vi "ConvertGoop2ToGoop3.vi"() -> (0 "error out":errorcluster)   [LabVIEW 2020]
uses:
  ConvertGoop2ToGoop3_SubVIs/ConvertGoop2ToGoop3_ClassInfo.ctl
  LvClass_class/GDSLvCLass_ClassSettingsType.ctl
  LvClass_class/GDSLvClass_PlugIn.ctl
  LvClass_class/GDSLvClass_PlugInTypes.ctl
  <vilib>/Utility/miscctls.llb/LVPositionTypeDef.ctl
  <vilib>/Utility/error.llb/DialogType.ctl
  <vilib>/picture/picture.llb/imagedata.ctl
  Provider_EndevoGOOP300/Templates/EndevoTemplateNames.ctl
  Provider_EndevoGOOP300/EndevoProviderName.ctl
  <vilib>/regexp/Match Regular Expression.xnode
panel:
  in  "Cancel":bool
  in  "Next":bool
  out "Tab":T1(tab)
  in  "Current GOOP2 top directory":path
  out "Additional VIs that has been found\nand will be relinked:":i32
  out "GOOP2 classes found":string
  in  "VisToRelink":path[](array[path])
  in  "Project":path caption="This project will be created and have all classes added to it:"
  in  "Progress":i32(listbox)
  in  "Done":bool
  out "State":string
  # "1."
  # "Select Top folder to start a recursive search for GOOP2 classes and application VIs."
  # "2."
  # "These classes\nhave been found.\n\nDo you want to convert them?"
  # "3."
  # "Have you backed up all your VIs in the selected folder?"
  # "Have you checked that all files in\nthe selected folder are writeable?"
  # "Relinking VIs outside top folder?\nIf you want to relink any VIs to the new classes that are outside the selected top folder, add them to the list below"
  # "4."
  # "Save VI dialog boxes!?!\nIt might pop up dialog boxes that asks you to save VIs that will be unloaded from memory, JUST press cancel for those."
  # "5."
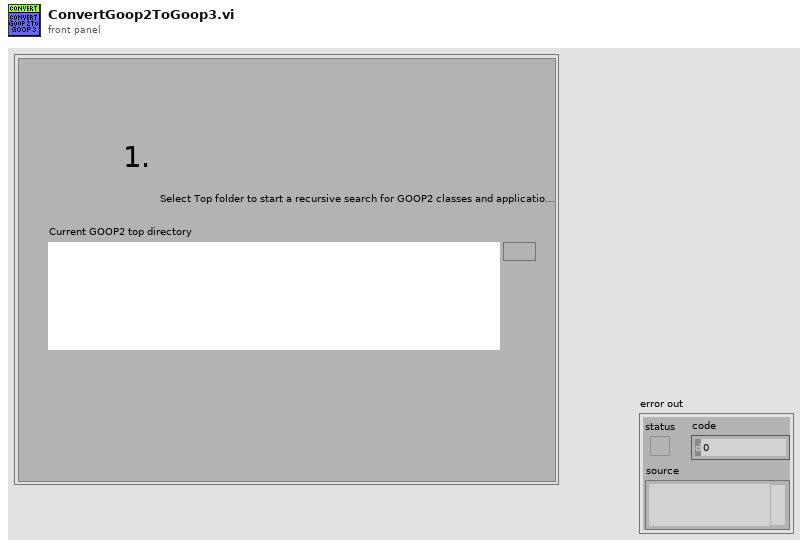
[diagram p1: front panel]
types:
  T1 = enum32{"GOOP2Dir", "ClassesFound", "BackedUp", "Start?", "Converting"}
  T2 = typedef "ConvertGoop2ToGoop3_ClassInfo.ctl" = cluster{"NoOfInheritance":i32, "LvClassPath":path, "ClassName":string, "ClassPrefix":string, "IsLLB":bool, "ClassFolder":path, "ViRefs":refnum<vi>[], "ClassRef":refnum<vi>, "InheritsFrom":path, "RootClass":path, "ViPathes":path[], "AllInheritanceClasses":string[], "TemplateVersionUsed":string, "UsingClassAttributes":bool, "ClassSettings":T3, "HeaderIcon":u8[][]}
  T3 = typedef "GDSLvCLass_ClassSettingsType.ctl" = cluster{"ClassProviderName":string, "ClassTemplateUsed":string, "ClassTemplateVersion":string, "ClassDescription":string, "PlugIns":T4[], "ConnectorPanePattern":string}
  T4 = typedef "GDSLvClass_PlugIn.ctl" = cluster{"Type":T5, "ID":string, "Version":string, "Path":path, "Name":string, "Data":variant}
  T5 = typedef "GDSLvClass_PlugInTypes.ctl" = enum16{"DesignPattern", "MethodTypes"}
  T6 = typedef "LVPositionTypeDef.ctl" = cluster{"Left":i32, "Top":i32}
  T7 = cluster{"TopFolderPath":path, "Classes":T2[], "SetToDynamicDispatch":refnum<vi>[], "error":errorcluster, "Project":path, "ProjectRef":refnum<vi>, "My Computer":refnum<vi>, "AppRef":refnum<vi>, "VIsToRelink":refnum<vi>[], "VIsToRelink(Paths)":path[], "CallParentMethod":cluster{"VIRef":refnum<vi>, "Position":T6}[], "TemplateVersionUsed":string}
  T8 = enum32{"GOOP2Dir", "ClassesFound", "GOOP3Dir", "Start?", "Converting"}
  T9 = typedef "imagedata.ctl" = cluster{"image type":i32, "image depth":i32, "image":u8[], "mask":u8[], "colors":u32[], "Rectangle":cluster{"left":i16, "top":i16, "right":i16, "bottom":i16}}
  T10 = typedef "EndevoTemplateNames.ctl" = enum16{"BaseTemplate", "SubTemplate", "BaseTemplate_4x4x4", "SubTemplate_4x4x4", "SingletonTemplate"}
  T11 = typedef "EndevoProviderName.ctl" = enum16{"EndevoGOOP300"}
  T12 = typedef "DialogType.ctl" = u16
  T13 = enum32{"invalid VI type", "Standard VI", "Control VI", "Global VI", "Polymorphic VI", "Configuration VI", "SubSystem", "Facade VI", "Method VI", "Statechart Diagram VI"}
  T14 = enum16{"Invalid Wire Rule", "Required", "Recommended", "Optional", "Dynamic Dispatch"}
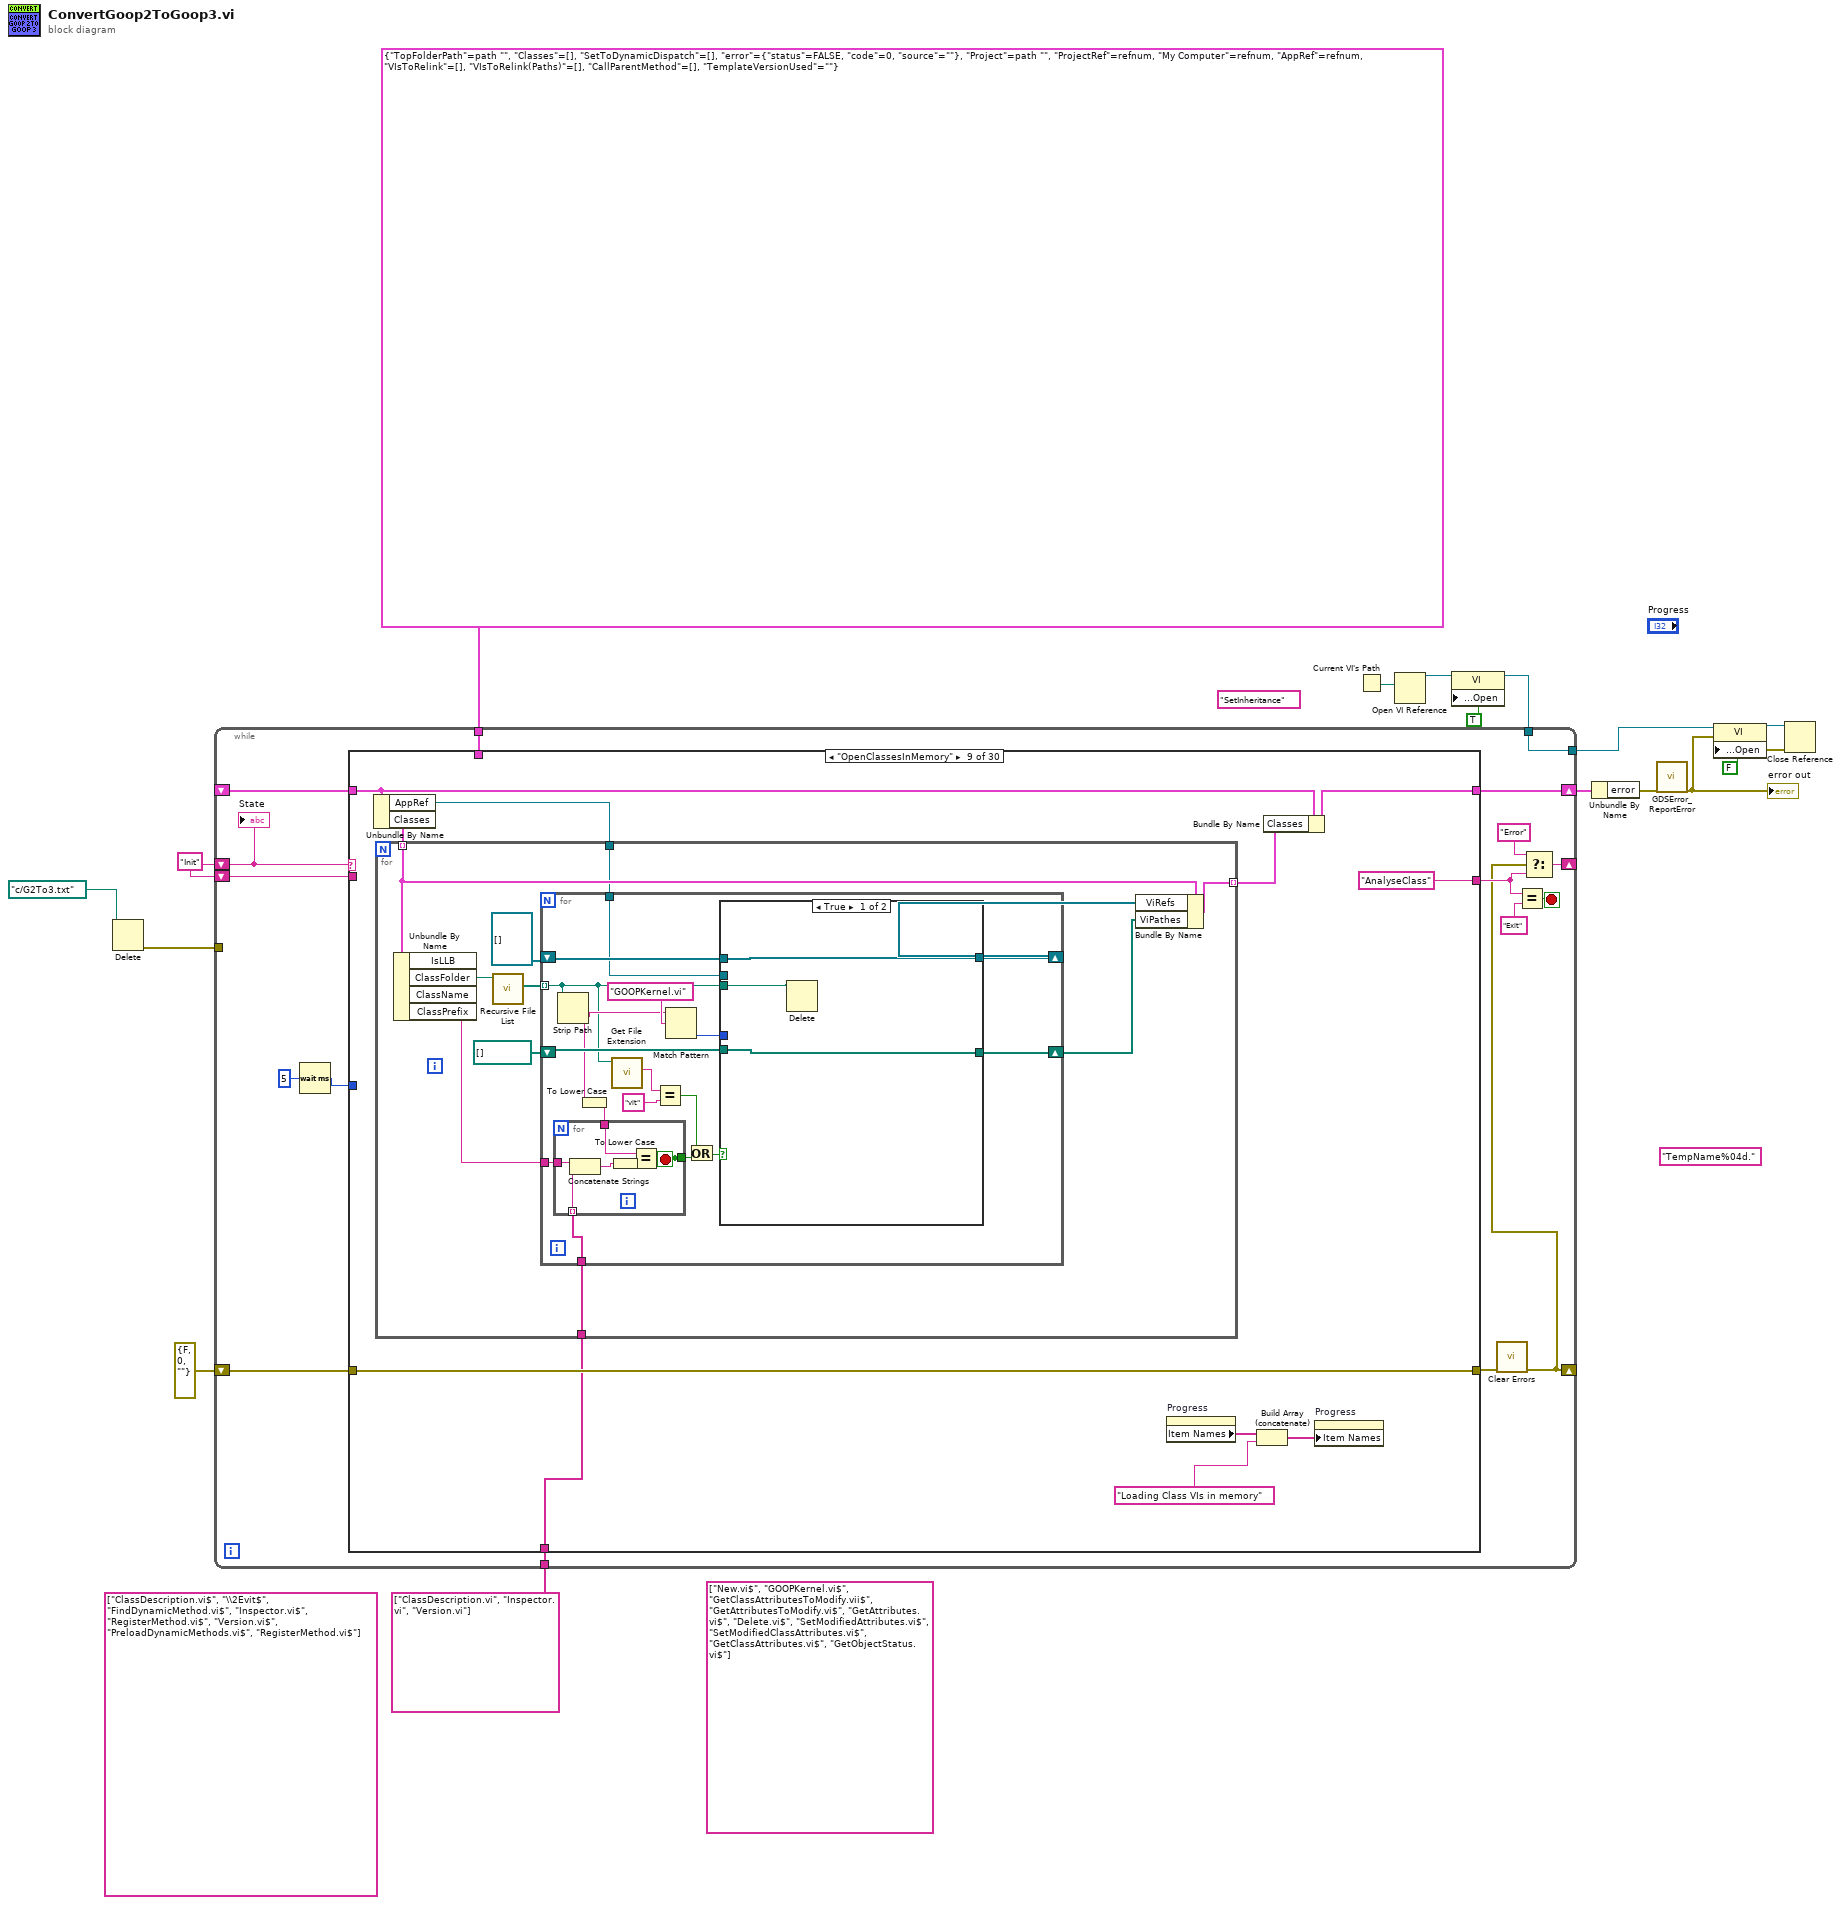
[diagram p0: block diagram]
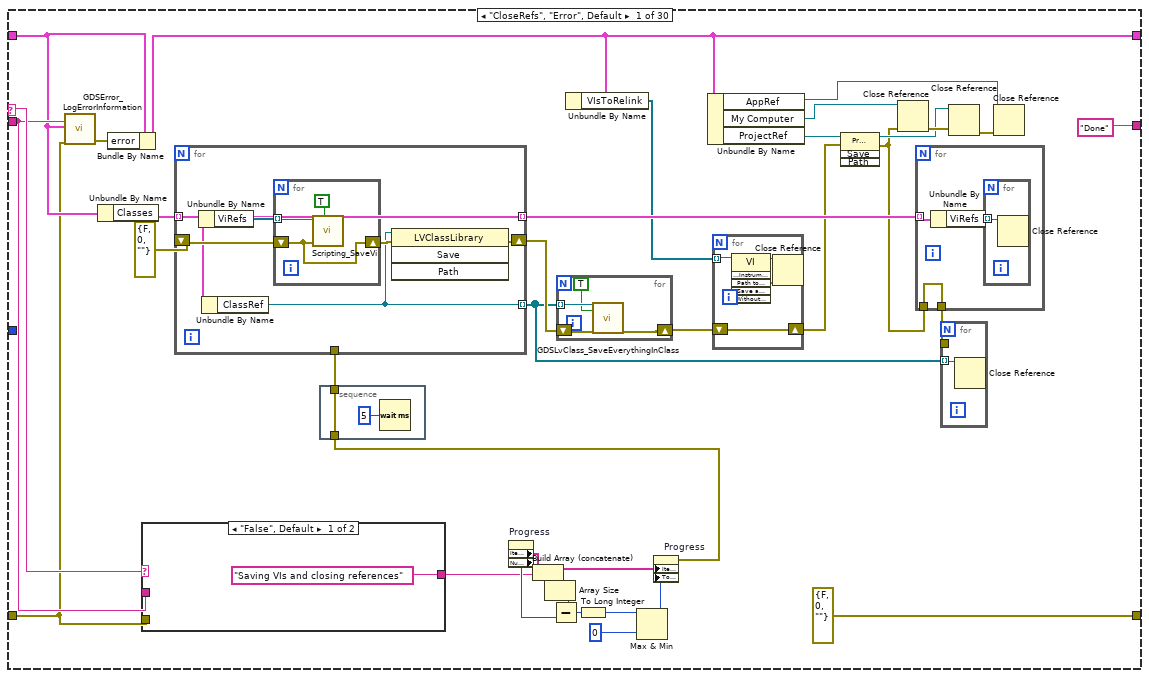
[diagram p2: hidden frame]
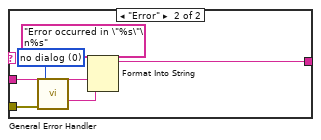
[diagram p3: hidden frame]
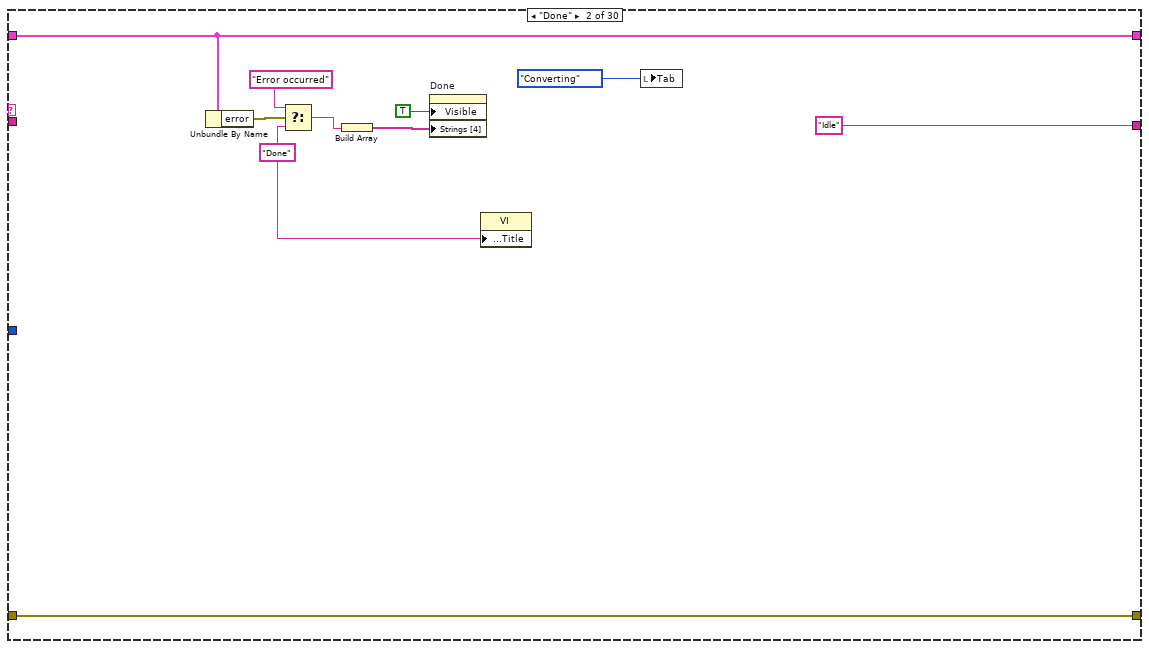
[diagram p4: hidden frame]
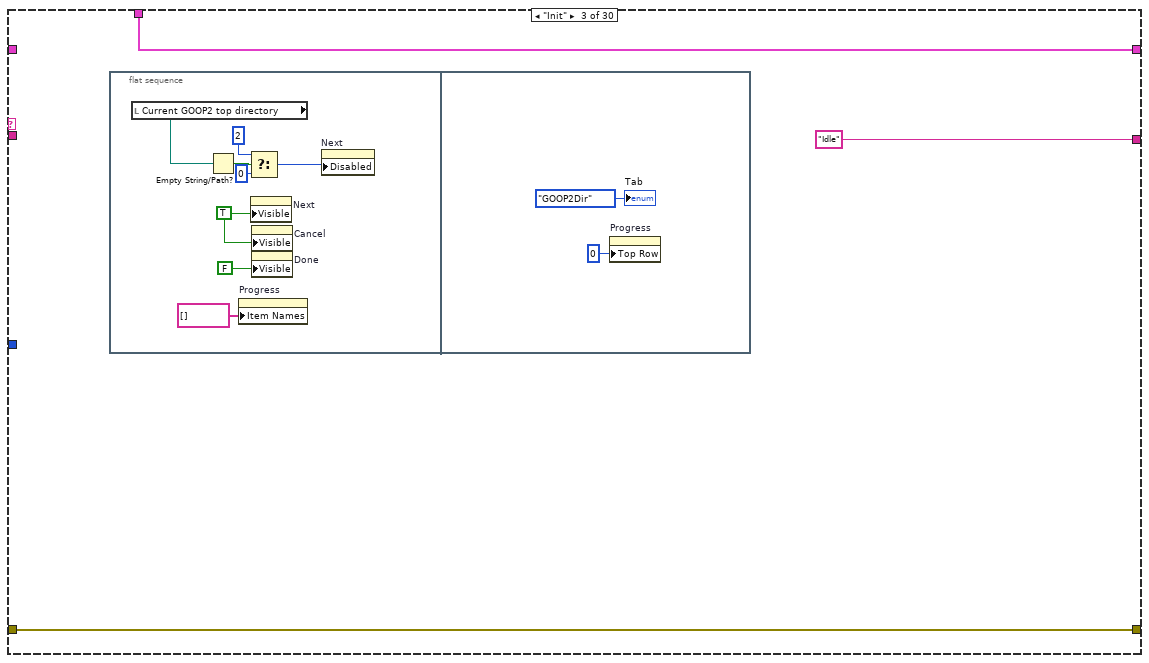
[diagram p5: hidden frame]
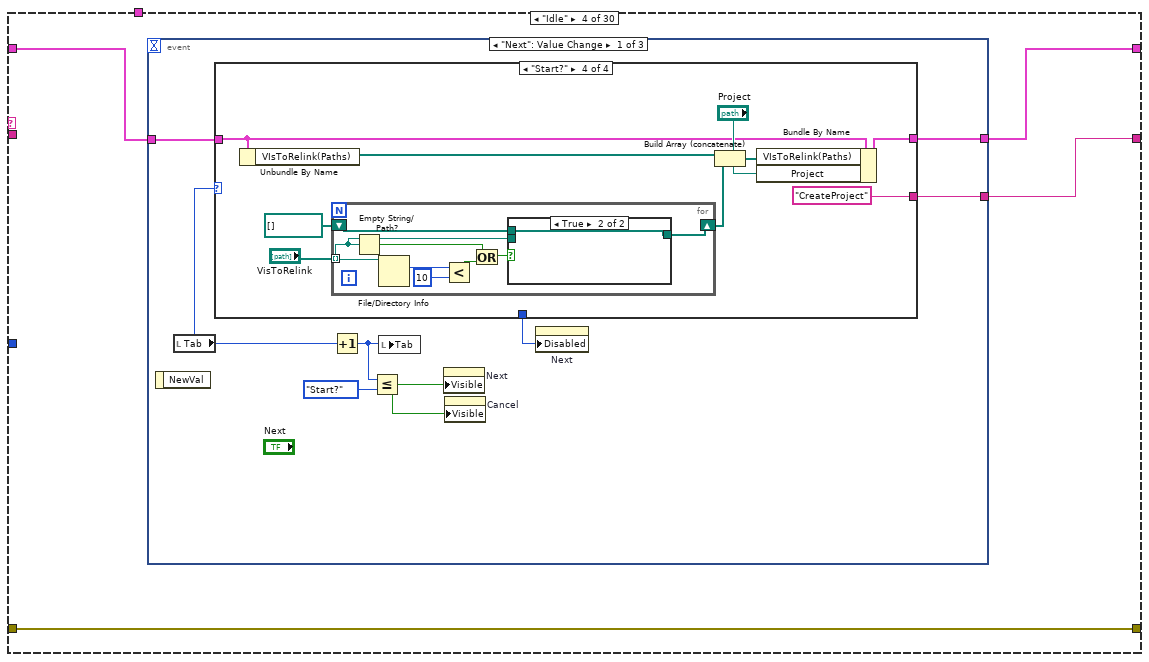
[diagram p6: hidden frame]
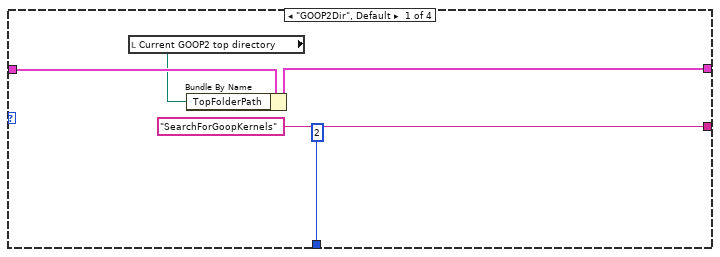
[diagram p7: hidden frame]
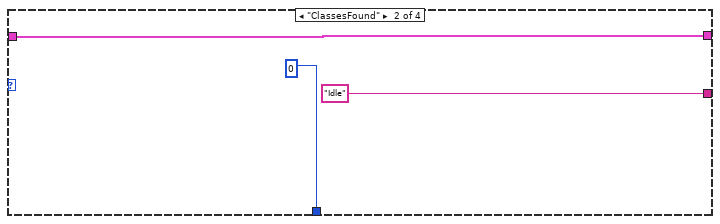
[diagram p8: hidden frame]
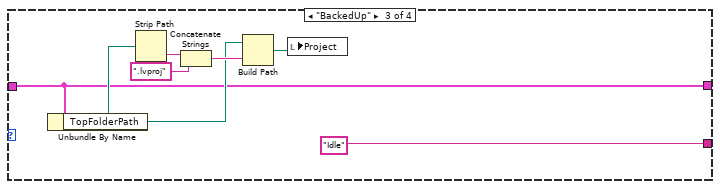
[diagram p9: hidden frame]
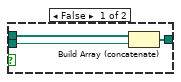
[diagram p10: hidden frame]
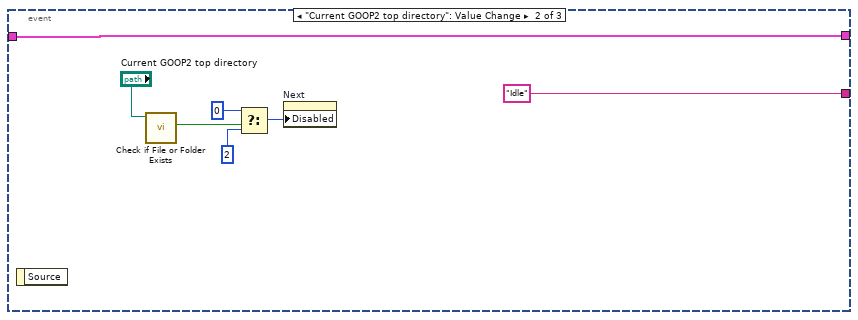
[diagram p11: hidden frame]
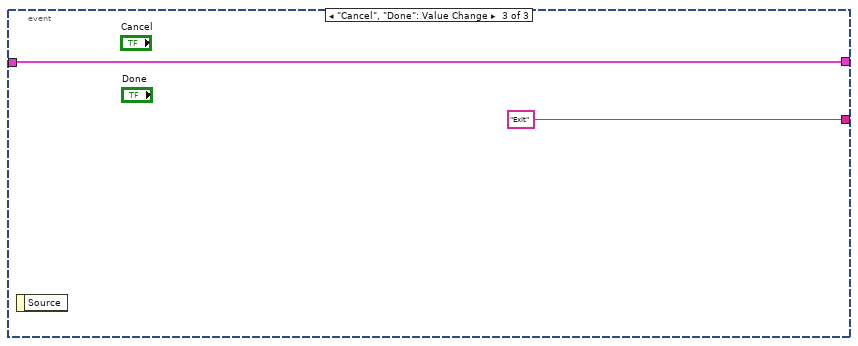
[diagram p12: hidden frame]
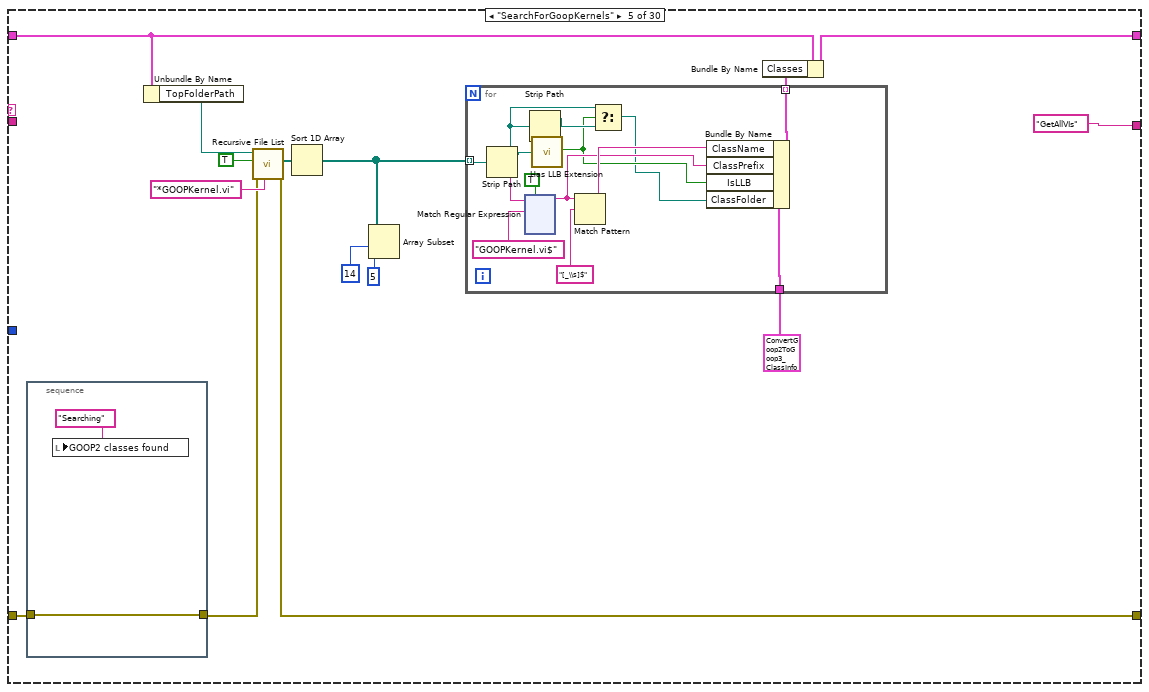
[diagram p13: hidden frame]
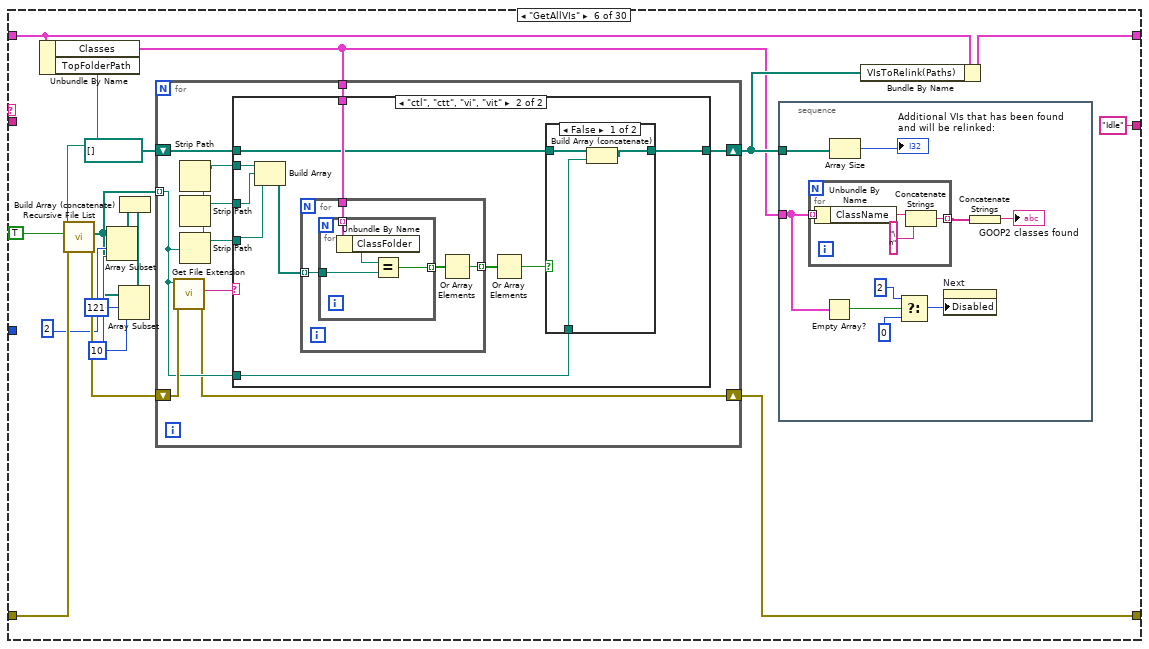
[diagram p14: hidden frame]
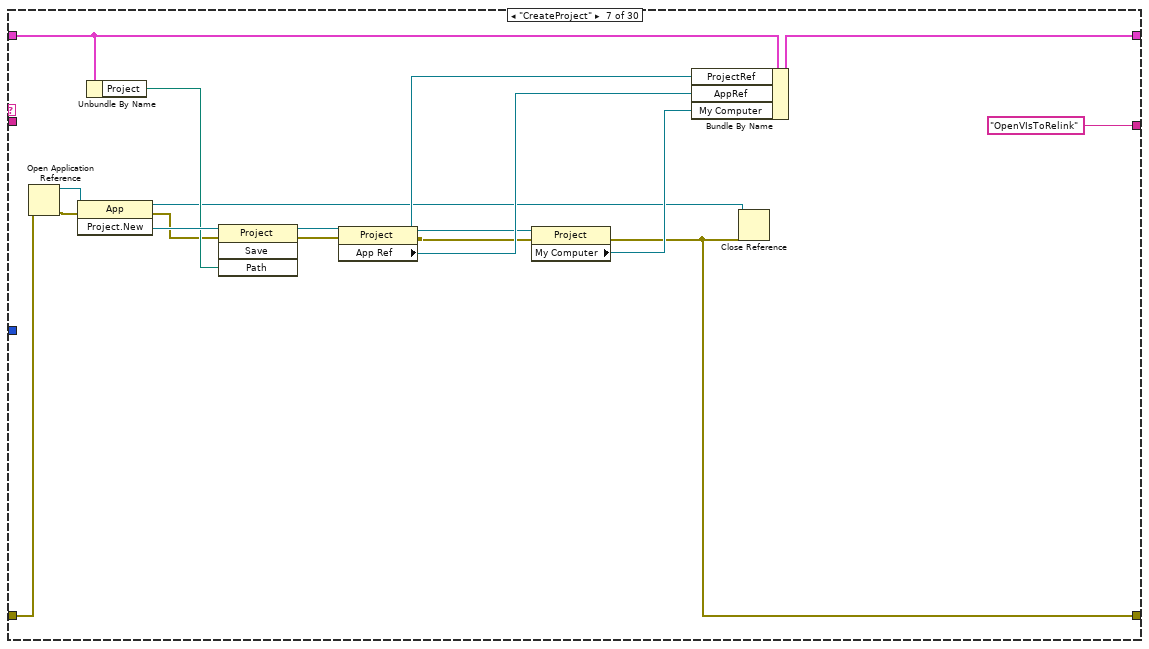
[diagram p17: hidden frame]
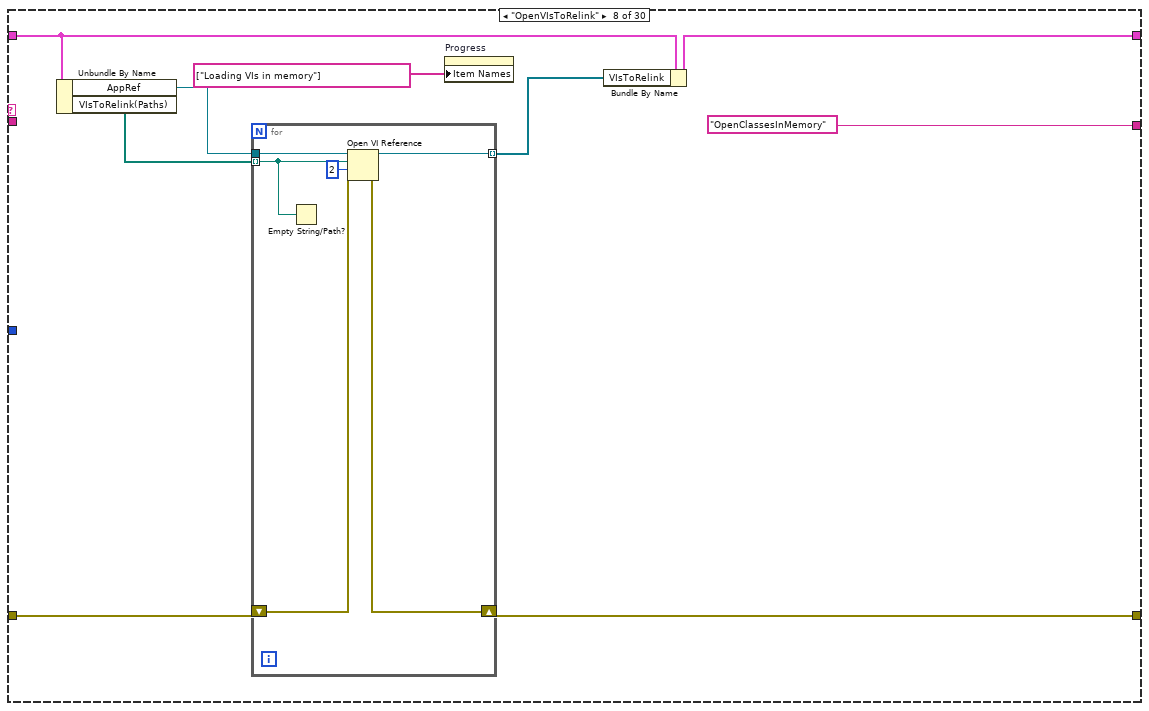
[diagram p18: hidden frame]
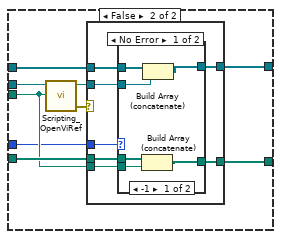
[diagram p19: hidden frame]
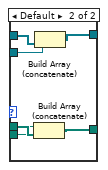
[diagram p20: hidden frame]
diagram:
  (unwired) "SetInheritance"
  (unwired) "TempName%04d." ("format string")
  (unwired) string[] ["ClassDescription.vi$", "\\2Evit$", "FindDynamicMethod.vi$", "Inspector.vi$", "RegisterMethod.vi$", "Version.vi$", "PreloadDynamicMethods.vi$", "RegisterMethod.vi$"] ("file names")
  (unwired) string[] ["New.vi$", "GOOPKernel.vi$", "GetClassAttributesToModify.vii$", "GetAttributesToModify.vi$", "GetAttributes.vi$", "Delete.vi$", "SetModifiedAttributes.vi$", "SetModifiedClassAttributes.vi$", "GetClassAttributes.vi$", "GetObjectStatus.vi$"] ("file names")
  w15 = "Init"
  n1 = Delete(path (use dialog)=path "c:/G2To3.txt" ("file (use dialog)")) -> (error out=w12:errorcluster)  [unwired: 4 in, 2 out]
  n2 = Current VI's Path() -> (path=w10:path)
  n3 = Open VI Reference(vi path=w10) -> (vi reference=w8:refnum<vi>)  [unwired: 5 in, 1 out]
  n4 = property class="VI"(reference=w8, "Front Panel.Open"=TRUE ("Front Panel Window:Open")) -> (reference out=w7:refnum<vi>)  [unwired: 1 in, 1 out]
  n5 = while {
    shift-right: [w19] -> _
    shift-left: errorcluster {"status"=FALSE, "code"=0, "source"=""} ("error IO") -> [w34]
    shift-right: [w33] -> _
    shift-left: w15 -> [w24]
    shift-right: [w28] -> w14
    shift-left: _ -> [w27]
    tunnel: T7 {"TopFolderPath"=path "", "Classes"=[], "SetToDynamicDispatch"=[], "error"={"status"=FALSE, "code"=0, "source"=""}, "Project"=path "", "ProjectRef"=refnum, "My Computer"=refnum, "AppRef"=refnum, "VIsToRelink"=[], "VIsToRelink(Paths)"=[], "CallParentMethod"=[], "TemplateVersionUsed"=""} -> [w26]
    shift-left: w15 -> [w25]
    tunnel: w12 -> [_]
    tunnel: w7 -> [w21]
    tunnel: [w21] -> w5
    tunnel: string[] ["ClassDescription.vi", "Inspector.vi", "Version.vi"] ("file names") -> [w18]
    stop <- w32 stop-if-true
    n6 = Wait (ms)(milliseconds to wait=u32 5) -> (millisecond timer value=w22:u32)
    n7 = case shown="\"OpenClassesInMemory\"" w24 {
      selector: w24 -> [w64 _ _ _ _ _ _ _ _ _ _ _ _ _ _ _ _ _ _ _ _ _ _ _ _ _ _ _ _ _]
      tunnel: w34 -> [w58 w109 w112 w124 w188 w335 w395 w407 w423 w504 w533 w576 w586 w625 w757 w799 w883 w929 w981 w1030 w1071 w1158 w1220 w1277 w1329 w1409 w1423 w1481 w1515 w1559]
      tunnel: [errorcluster {"status"=FALSE, "code"=0, "source"=""} ("error IO") w109 w112 w124 w192 w333 w386 w406 w423 w504 w532 w574 w582 w626 w760 w798 w894 w931 w982 w1032 w1065 w1145 w1213 w1274 w1335 w1408 w1423 w1482 w1510 w1547] -> w20
      tunnel: ["Done" "Idle" "Idle" w125 "GetAllVIs" "Idle" "OpenVIsToRelink" "OpenClassesInMemory" "AnalyseClass" "RemoveReentrantForDynamicDispatchVIs" "RecompilingVIs" "AddVIsToProject" "RenameFiles" "RenameTempNames" "FindAllCallParentMethodCalls" "UpdateNewVI" "SetInheritance" "UpdateLvClassIcon" "UpdateLvClassAttributes" "UpdateUtilsVIs" "UpdateSubClassKernels" "UpdateVIsGoopRefs" "UpdateCreate" "UpdateDynamicDispatchVIs" "ExtraSave" "SetDynamicDispatch" "UpdateAllCallParentMethods" "UpdateDestroy" "UpdateClassInfo" "CloseRefs"] -> w29
      tunnel: [w47 w108 w111 w126 w190 w331 w397 w409 w425 w502 w534 w575 w579 w624 w758 w796 w881 w930 w984 w1031 w1067 w1144 w1212 w1271 w1332 w1407 w1422 w1479 w1514 w1558] -> w28
      tunnel: w27 -> [w60 w108 _ w127 w191 w332 w399 w410 w426 w503 w534 w575 w579 w619 w758 w797 w881 w930 w984 w1031 w1064 w1144 w1212 w1271 w1327 w1407 w1422 w1479 w1514 w1558]
      tunnel: w26 -> [_ _ w111 _ _ _ _ _ _ _ _ _ _ _ _ _ _ _ _ _ _ _ _ _ _ _ _ _ _ _]
      tunnel: w25 -> [w63 _ _ _ _ _ _ _ _ _ _ _ _ _ _ _ _ _ _ _ _ _ _ _ _ _ _ _ _ _]
      tunnel: w22 -> [_ _ _ _ _ _ _ _ _ _ _ _ _ _ _ _ _ _ _ _ _ _ _ _ _ _ _ _ _ _]
      tunnel: w18 -> [_ _ _ _ _ _ _ _ w417 _ _ _ _ _ _ _ _ _ _ _ _ _ _ _ _ _ _ _ _ _]
      frame "CloseRefs", "Error", Default {
        n8 = call "GDSError_LogErrorInformation.vi"("State"=w63, "LocalVariableData"=w60, "error in (no error)"=w58) -> ("error out"=w50:errorcluster)  [unwired: 16 in]
        n9 = Unbundle By Name(w60) -> ("Classes"=w68:T2[])
        n10 = Bundle By Name(cluster=w60, "error"=w50) -> (w47:T7)
        n11 = case shown="\"False\", Default" w64 {
          tunnel: w63 -> [_ w81]
          tunnel: w58 -> [_ w79]
          tunnel: ["Saving VIs and closing references" w77] -> w37
          frame "False", Default {
          }
          frame "Error" {
            w80 = T12 0 items=["no dialog", "OK message", "continue or stop message", "OK message + warnings", "continue/stop + warnings"] ("type of dialog (OK msg:1)")
            n12 = call <vilib>:"General Error Handler.vi"("type of dialog (OK msg:1)"=w80, "error in (no error)"=w79) -> ("message"=w78:string)  [unwired: 9 in, 4 out]
            n13 = Format Into String(format string="Error occurred in \"%s\"\n%s", w81, w78) -> (resulting string=w77:string)  [unwired: 2 in, 1 out]
          }
        }
        n14 = property on="Progress" class="LstBox (strict)"() -> ("Item Names"=w45:string[], "Number of Rows"=w39:u32)  [unwired: 2 in, 2 out]
        n15 = Build Array (concatenate)(w45, w37) -> (w40:string[])
        n16 = Array Size(array=w40) -> (size(s)=w44:i32)
        n17 = Subtract(x=w44, y=w39) -> (x-y=w43:u32)
        n18 = Unbundle By Name(w47) -> ("VIsToRelink"=w52:refnum<vi>[])
        n19 = To Long Integer(number=w43) -> (32bit integer=w41:i32)
        n20 = Max & Min(x=w41, y=0) -> (max(x,y)=w38:i32)  [unwired: 1 out]
        n21 = property on="Progress" class="LstBox (strict)"("Item Names"=w40, "Top Row"=w38) -> (error out=w36:errorcluster)  [unwired: 2 in, 1 out]
        n22 = stacked-sequence {
          tunnel: w36 -> [w70]
          tunnel: [w70] -> w35
          frame #0 {
            n23 = Wait (ms)(milliseconds to wait=u32 5) -> ()  [unwired: 1 out]
          }
        }
        n24 = for {
          tunnel: w68 -> [w95] mode=indexing
          tunnel: [w95] -> w67 mode=indexing
          shift-right: [w93] -> w66
          shift-left: errorcluster {"status"=FALSE, "code"=0, "source"=""} ("error out") -> [w96]
          tunnel: [w92] -> w65 mode=indexing
          tunnel: w35 -> [_]
          n25 = Unbundle By Name(w95) -> ("ViRefs"=w97:refnum<vi>[])
          n26 = Unbundle By Name(w95) -> ("ClassRef"=w92:refnum<vi>)
          n27 = for {
            tunnel: w97 -> [w100] mode=indexing
            shift-right: [w98] -> w94
            shift-left: w96 -> [w98]
            n28 = call "Scripting_SaveVi.vi"("ForceResaving(False)"=TRUE, "error in (no error)"=w98, "VIRefToSaveIn"=w100) -> ()  [unwired: 7 in, 2 out]
          }
          n29 = invoke class="LVClassLibrary" method="Save"(reference=w92, error in=w94) -> (error out=w93:errorcluster)  [unwired: 2 in, 3 out]
        }
        n30 = for {
          shift-right: [w86] -> w49
          shift-left: w66 -> [w87]
          tunnel: w65 -> [w85] mode=indexing
          n31 = call "GDSLvClass_SaveEverythingInClass.vi"("ClassRefIn"=w85, "ForceResaving(False)"=TRUE, "error in"=w87) -> ("error out"=w86:errorcluster)  [unwired: 15 in, 1 out]
        }
        n32 = Unbundle By Name(w47) -> ("AppRef"=w53:refnum<vi>, "My Computer"=w46:refnum<vi>, "ProjectRef"=w57:refnum<vi>)
        n33 = for {
          tunnel: w52 -> [w73] mode=indexing
          shift-right: [w72] -> w48
          shift-left: w49 -> [w72]
          n34 = invoke class="VI" method="Save.Instrument"(reference=w73) -> (reference out=w74:refnum<vi>, error out=w75:errorcluster)  [unwired: 5 in, 4 out]
          n35 = Close Reference(reference=w74, error in (no error)=w75) -> ()  [unwired: 1 out]
        }
        n36 = invoke class="Project" method="Save"(reference=w57, error in=w48) -> (reference out=w55:refnum<vi>, error out=w51:errorcluster)  [unwired: 2 in, 2 out]
        n37 = Close Reference(reference=w46, error in (no error)=w51) -> (error out=w56:errorcluster)
        n38 = for {
          tunnel: w67 -> [w90] mode=indexing
          tunnel: w51 -> [w88]
          tunnel: [w88] -> w62
          n39 = Unbundle By Name(w90) -> ("ViRefs"=w89:refnum<vi>[])
          n40 = for {
            tunnel: w89 -> [w91] mode=indexing
            n41 = Close Reference(reference=w91) -> ()  [unwired: 1 in, 1 out]
          }
        }
        n42 = for {
          tunnel: w65 -> [w83] mode=indexing
          tunnel: w62 -> [_]
          n43 = Close Reference(reference=w83) -> ()  [unwired: 1 in, 1 out]
        }
        n44 = Close Reference(reference=w55, error in (no error)=w56) -> (error out=w54:errorcluster)
        n45 = Close Reference(reference=w53, error in (no error)=w54) -> ()  [unwired: 1 out]
      }
      frame "Done" {
        w101 = "Done"
        n46 = Unbundle By Name(w108) -> ("error"=w107:errorcluster)
        n47 = Select(t="Error occurred", s=w107, f=w101) -> (s? t:f=w104:string)
        n48 = Build Array(w104) -> (w103:string[])
        n49 = property on="Done" class="Bool"("Visible"=TRUE, "Strings [4]"=w103) -> ()  [unwired: 2 in, 2 out]
        n50 = property class="VI"("Front Panel.Title"=w101) -> ()  [unwired: 2 in, 2 out]
        n51 = local write "Tab"(T1."Converting" ("Tab")) -> ()
      }
      frame "Init" {
        n52 = flat-sequence {
          frame #0 {
            w121 = TRUE ("Visible")
            n53 = local read "Current GOOP2 top directory"() -> (w118:path)
            n54 = Empty String/Path?(string/path=w118) -> (empty?=w117:bool)
            n55 = property on="Progress" class="LstBox (strict)"("Item Names"=string[] []) -> ()  [unwired: 2 in, 2 out]
            n56 = Select(t=u8 2 ("Disabled"), s=w117, f=u8 0) -> (s? t:f=w115:u8)
            n57 = property on="Next" class="Bool"("Visible"=w121) -> ()  [unwired: 2 in, 2 out]
            n58 = property on="Cancel" class="Bool"("Visible"=w121) -> ()  [unwired: 2 in, 2 out]
            n59 = property on="Done" class="Bool"("Visible"=FALSE) -> ()  [unwired: 2 in, 2 out]
            n60 = property on="Next" class="Bool"("Disabled"=w115) -> ()  [unwired: 2 in, 2 out]
          }
          frame #1 {
            n61 = property on="Progress" class="LstBox (strict)"("Top Row"=0) -> ()  [unwired: 2 in, 2 out]
            "Tab" <- T1."GOOP2Dir" ("Tab")
          }
        }
      }
      frame "Idle" {
        n62 = event shown="[0] \"Next\": Value Change" {
          selector: _ -> [_ _ _]
          dyn-events: _ -> [_ _ _]
          timeout: _ -> [_ _ _]
          tunnel: w127 -> [w131 w174 w179]
          tunnel: [w130 w174 w179] -> w126
          tunnel: [w129 "Idle" "Exit"] -> w125
          event "Next": Value Change {
            n63 = event-data() -> ()  [unwired: 1 in, 1 out]
            n64 = local read "Tab"() -> (w132:T1)
            n65 = case shown="\"Start?\"" w132 {
              tunnel: w131 -> [w140 w142 w145 w156]
              tunnel: [w139 w142 w145 w159] -> w130
              tunnel: ["SearchForGoopKernels" "Idle" "Idle" "CreateProject"] -> w129
              tunnel: [u8 2 ("Disabled") u8 0 ("f") _ _] -> w128
              frame "GOOP2Dir", Default {
                n66 = local read "Current GOOP2 top directory"() -> (w137:path)
                n67 = Bundle By Name(cluster=w140, "TopFolderPath"=w137) -> (w139:T7)
              }
              frame "ClassesFound" {
              }
              frame "BackedUp" {
                n68 = Unbundle By Name(w145) -> ("TopFolderPath"=w146:path)
                n69 = Strip Path(path=w146) -> (name=w149:string)  [unwired: 1 out]
                n70 = Concatenate Strings(w149, ".lvproj" ("string")) -> (w147:string)
                n71 = Build Path(base path=w146, name or relative path=w147) -> (appended path=w144:path)
                n72 = local write "Project"(w144) -> ()
              }
              frame "Start?" {
                n73 = Unbundle By Name(w156) -> ("VIsToRelink(Paths)"=w155:path[])
                n74 = for {
                  tunnel: "VisToRelink" -> [w161] mode=indexing
                  shift-right: [w160] -> w151
                  shift-left: path[] [] -> [w162]
                  n75 = Empty String/Path?(string/path=w161) -> (empty?=w164:bool)
                  n76 = File/Directory Info(path=w161) -> (size=w167:i64)  [unwired: 1 in, 6 out]
                  n77 = Less?(x=w167, y=i64 10) -> (x < y?=w165:bool)
                  n78 = Or(x=w164, y=w165) -> (x .or. y?=w163:bool)
                  n79 = case shown="True" w163 {
                    tunnel: w162 -> [w170 w171]
                    tunnel: w161 -> [w169 _]
                    tunnel: [w168 w171] -> w160
                    frame False {
                      n80 = Build Array (concatenate)(w170, w169) -> (w168:path[])
                    }
                    frame True {
                    }
                  }
                }
                n81 = Build Array (concatenate)(w155, w151) -> (w154:path[])
                n82 = Bundle By Name(cluster=w156, "VIsToRelink(Paths)"=w154, "Project"="Project") -> (w159:T7)
              }
            }
            n83 = Increment(x=w132) -> (x+1=w135:T1)
            n84 = Less Or Equal?(x=w135, y=T8."Start?") -> (x <= y?=w133:bool)
            n85 = local write "Tab"(w135) -> ()
            n86 = property on="Next" class="Bool"("Visible"=w133) -> ()  [unwired: 2 in, 2 out]
            n87 = property on="Cancel" class="Bool"("Visible"=w133) -> ()  [unwired: 2 in, 2 out]
            n88 = property on="Next" class="Bool"("Disabled"=w128) -> ()  [unwired: 2 in, 2 out]
          }
          event "Current GOOP2 top directory": Value Change {
            n89 = event-data() -> ()  [unwired: 1 in, 1 out]
            n90 = call <vilib>:"Check if File or Folder Exists.vi"("path"="Current GOOP2 top directory") -> ("file or folder exists?"=w178:bool)  [unwired: 8 in, 2 out]
            n91 = Select(t=u8 0, s=w178, f=u8 2 ("Disabled")) -> (s? t:f=w177:u8)
            n92 = property on="Next" class="Bool"("Disabled"=w177) -> ()  [unwired: 2 in, 2 out]
          }
          event "Cancel", "Done": Value Change {
            n93 = event-data() -> ()  [unwired: 1 in, 1 out]
          }
        }
      }
      frame "SearchForGoopKernels" {
        n94 = stacked-sequence {
          tunnel: w188 -> [w196]
          tunnel: [w196] -> w187
          frame #0 {
            n95 = local write "GOOP2 classes found"("Searching" ("GOOP2 classes found")) -> ()
          }
        }
        n96 = Unbundle By Name(w191) -> ("TopFolderPath"=w195:path)
        n97 = call <vilib>:"Recursive File List.vi"("pattern"="*GOOPKernel.vi", "error in (no error)"=w187, "Treat LLBs as Folders?"=TRUE, "Folder Path"=w195) -> ("error out"=w192:errorcluster, "All Files in Dir"=w186:path[])  [unwired: 3 in, 3 out]
        n98 = Sort 1D Array(array=w186) -> (sorted array=w182:path[])
        n99 = Array Subset(array=w182, index=14, length=5) -> ()  [unwired: 1 out]
        n100 = for {
          tunnel: w182 -> [w210] mode=indexing
          tunnel: T2 {"NoOfInheritance"=0, "LvClassPath"=path "", "ClassName"="", "ClassPrefix"="", "IsLLB"=FALSE, "ClassFolder"=path "", "ViRefs"=[], "ClassRef"=refnum, "InheritsFrom"=path "", "RootClass"=path "", "ViPathes"=[], "AllInheritanceClasses"=[], "TemplateVersionUsed"="", "UsingClassAttributes"=FALSE, "ClassSettings"={"ClassProviderName"="", "ClassTemplateUsed"="", "ClassTemplateVersion"="", "ClassDescription"="", "PlugIns"=[], "ConnectorPanePattern"=""}, "HeaderIcon"=[]} ("output cluster") -> [w203]
          tunnel: [w198] -> w181 mode=indexing
          n101 = Strip Path(path=w210) -> (stripped path=w205:path, name=w209:string)
          n102 = xnode "Match Regular Expression"("input string"=w209, "regular expression"="GOOPKernel.vi$", "ignore case? (F)"=TRUE) -> ("before match"=w201:string)  [unwired: 3 in, 4 out]
          n103 = Strip Path(path=w205) -> (stripped path=w204:path)  [unwired: 1 out]
          n104 = call <vilib>:"Has LLB Extension.vi"("path"=w205) -> ("path to VI library?"=w200:bool)
          n105 = Match Pattern(string=w201, regular expression="[_\\s]$") -> (before substring=w202:string)  [unwired: 1 in, 3 out]
          n106 = Select(t=w205, s=w200, f=w204) -> (s? t:f=w199:path)
          n107 = Bundle By Name(cluster=w203, "ClassName"=w202, "ClassPrefix"=w201, "IsLLB"=w200, "ClassFolder"=w199) -> (w198:T2)
        }
        n108 = Bundle By Name(cluster=w191, "Classes"=w181) -> (w190:T7)
      }
      frame "GetAllVIs" {
        w326 = 10 ("length")
        n109 = Unbundle By Name(w332) -> ("Classes"=w329:T2[], "TopFolderPath"=w338:path)
        n110 = call <vilib>:"Recursive File List.vi"("error in (no error)"=w335, "Treat LLBs as Folders?"=TRUE, "Folder Path"=w338) -> ("error out"=w334:errorcluster, "All Files in Dir"=w322:path[])  [unwired: 4 in, 3 out]
        n111 = Array Subset(array=w322, index=2, length=w326) -> (w324:path[])
        n112 = Array Subset(array=w322, index=121, length=w326) -> (w323:path[])
        n113 = Build Array (concatenate)(w324, w323) -> ()  [unwired: 1 out]
        n114 = for {
          shift-right: [w360] -> w330
          shift-left: path[] [] ("All Files in Dir") -> [w359]
          tunnel: w322 -> [w353] mode=indexing
          shift-right: [w352] -> w333
          shift-left: w334 -> [w358]
          tunnel: w329 -> [w354]
          n115 = call <vilib>:"Get File Extension.vi"("error in (no error)"=w358, "file"=w353) -> ("error out"=w352:errorcluster, "lowercase file extension"=w361:string)  [unwired: 5 in, 3 out]
          n116 = Strip Path(path=w353) -> (stripped path=w357:path)  [unwired: 1 out]
          n117 = Strip Path(path=w357) -> (stripped path=w355:path)  [unwired: 1 out]
          n118 = Strip Path(path=w355) -> (stripped path=w356:path)  [unwired: 1 out]
          n119 = case shown="\"ctl\", \"ctt\", \"vi\", \"vit\"" w361 {
            tunnel: [w362 w365] -> w360
            tunnel: w359 -> [w362 w364]
            tunnel: w357 -> [_ w370]
            tunnel: w356 -> [_ w372]
            tunnel: w355 -> [_ w371]
            tunnel: w354 -> [_ w368]
            tunnel: w353 -> [_ w363]
            frame Default {
            }
            frame "ctl", "ctt", "vi", "vit" {
              n120 = Build Array(w372, w371, w370) -> (w369:path[])
              n121 = for {
                tunnel: w369 -> [w379] mode=indexing
                tunnel: w368 -> [w380]
                tunnel: [w377] -> w367 mode=indexing
                n122 = for {
                  tunnel: w380 -> [w384] mode=indexing
                  tunnel: w379 -> [w382]
                  tunnel: [w381] -> w378 mode=indexing
                  n123 = Unbundle By Name(w384) -> ("ClassFolder"=w383:path)
                  n124 = Equal?(x=w383, y=w382) -> (x = y?=w381:bool)
                }
                n125 = Or Array Elements(Boolean array=w378) -> (logical OR=w377:bool)
              }
              n126 = Or Array Elements(Boolean array=w367) -> (logical OR=w366:bool)
              n127 = case shown="False" w366 {
                tunnel: [w374 w376] -> w365
                tunnel: w364 -> [w375 w376]
                tunnel: w363 -> [w373 _]
                frame False {
                  n128 = Build Array (concatenate)(w375, w373) -> (w374:path[])
                }
                frame True {
                }
              }
            }
          }
        }
        n129 = stacked-sequence {
          tunnel: w329 -> [w339]
          tunnel: w330 -> [w341]
          frame #0 {
            n130 = for {
              tunnel: w339 -> [w351] mode=indexing
              tunnel: [w348] -> w347 mode=indexing
              n131 = Unbundle By Name(w351) -> ("ClassName"=w350:string)
              n132 = Concatenate Strings(w350, "\n" ("string")) -> (w348:string)
            }
            n133 = Empty Array?(array=w339) -> (empty?=w342:bool)
            n134 = Array Size(array=w341) -> (size(s)=→"Additional VIs that has been found\nand will be relinked:":i32)
            n135 = Select(t=u8 2, s=w342, f=u8 0 ("Disabled")) -> (s? t:f=w345:u8)
            n136 = property on="Next" class="Bool"("Disabled"=w345) -> ()  [unwired: 2 in, 2 out]
            n137 = Concatenate Strings(w347) -> (→"GOOP2 classes found":string)
          }
        }
        n138 = Bundle By Name(cluster=w332, "VIsToRelink(Paths)"=w330) -> (w331:T7)
      }
      frame "CreateProject" {
        n139 = Open Application Reference(8:w395) -> (0:w396:errorcluster, 3:w394:refnum<vi>)  [unwired: 3 in]
        n140 = invoke class="App" method="Project.New"(reference=w394, error in=w396) -> (reference out=w385:refnum<vi>, error out=w398:errorcluster, "Project:New"=w401:refnum<vi>)  [unwired: 1 in]
        n141 = Unbundle By Name(w399) -> ("Project"=w400:path)
        n142 = invoke class="Project" method="Save"(reference=w401, error in=w398, "Path"=w400) -> (reference out=w390:refnum<vi>, error out=w391:errorcluster)  [unwired: 1 in, 2 out]
        n143 = property class="Project"(reference=w390, error in=w391) -> (reference out=w389:refnum<vi>, error out=w388:errorcluster, "App Ref"=w392:refnum<vi>)
        n144 = property class="Project"(reference=w389, error in=w388) -> (error out=w386:errorcluster, "My Computer"=w387:refnum<vi>)  [unwired: 1 out]
        n145 = Bundle By Name(cluster=w399, "ProjectRef"=w389, "AppRef"=w392, "My Computer"=w387) -> (w397:T7)
        n146 = Close Reference(reference=w385, error in (no error)=w386) -> ()  [unwired: 1 out]
      }
      frame "OpenVIsToRelink" {
        n147 = Unbundle By Name(w410) -> ("AppRef"=w408:refnum<vi>, "VIsToRelink(Paths)"=w402:path[])
        n148 = for {
          tunnel: w408 -> [w416]
          shift-right: [w414] -> w406
          shift-left: w407 -> [w415]
          tunnel: [w413] -> w405 mode=indexing
          tunnel: w402 -> [w411] mode=indexing
          n149 = Empty String/Path?(string/path=w411) -> ()  [unwired: 1 out]
          n150 = Open VI Reference(application reference (local)=w416, vi path=w411, options=2, error in (no error)=w415) -> (vi reference=w413:refnum<vi>, error out=w414:errorcluster)  [unwired: 2 in]
        }
        n151 = property on="Progress" class="LstBox (strict)"("Item Names"=string[] ["Loading VIs in memory"]) -> ()  [unwired: 2 in, 2 out]
        n152 = Bundle By Name(cluster=w410, "VIsToRelink"=w405) -> (w409:T7)
      }
      frame "OpenClassesInMemory" {
        n153 = Unbundle By Name(w426) -> ("AppRef"=w421:refnum<vi>, "Classes"=w427:T2[])
        n154 = for {
          tunnel: w427 -> [w435] mode=indexing
          tunnel: [w433] -> w422 mode=indexing
          tunnel: w417 -> [w432]
          tunnel: w421 -> [w429]
          n155 = Unbundle By Name(w435) -> ("ClassFolder"=w438:path, "ClassPrefix"=w428:string)  [unwired: 2 out]
          n156 = call <vilib>:"Recursive File List.vi"("Folder Path"=w438) -> ("All Files in Dir"=w437:path[])  [unwired: 6 in, 4 out]
          n157 = for {
            tunnel: w437 -> [w444] mode=indexing
            shift-right: [w454] -> w434
            shift-left: refnum<vi>[] [] -> [w455]
            tunnel: w432 -> [w453]
            shift-right: [w451] -> w431
            shift-left: path[] [] -> [w452]
            tunnel: w429 -> [w450]
            tunnel: w428 -> [w446]
            n158 = Strip Path(path=w444) -> (name=w447:string)  [unwired: 1 out]
            n159 = To Lower Case(string=w447) -> (all lower case string=w445:string)
            n160 = for {
              tunnel: w445 -> [w461]
              tunnel: w453 -> [w459] mode=indexing
              tunnel: [w457] -> w440
              tunnel: w446 -> [w460]
              stop <- w457 stop-if-true
              n161 = Concatenate Strings(w460, w459) -> (w458:string)
              n162 = To Lower Case(string=w458) -> (all lower case string=w456:string)
              n163 = Equal?(x=w461, y=w456) -> (x = y?=w457:bool)
            }
            n164 = call <vilib>:"Get File Extension.vi"("file"=w444) -> ("lowercase file extension"=w442:string)  [unwired: 6 in, 4 out]
            n165 = Equal?(x=w442, y="vit") -> (x = y?=w441:bool)
            n166 = Match Pattern(string=w447, regular expression="GOOPKernel.vi") -> (offset past match=w448:i32)  [unwired: 1 in, 3 out]
            n167 = Or(x=w441, y=w440) -> (x .or. y?=w439:bool)
            n168 = case shown="True" w439 {
              tunnel: w444 -> [w462 w467]
              tunnel: w455 -> [w464 w471]
              tunnel: [w464 w470] -> w454
              tunnel: w452 -> [w463 w469]
              tunnel: [w463 w468] -> w451
              tunnel: w450 -> [_ w466]
              tunnel: w448 -> [_ w465]
              frame True {
                n169 = Delete(path (use dialog)=w462) -> ()  [unwired: 4 in, 3 out]
              }
              frame False {
                n170 = call "Scripting_OpenViRef.vi"("ViPath/ViName/Viref"=w467, "AppRef"=w466) -> ("error out"=w473:errorcluster, "vi reference"=w472:refnum<vi>)  [unwired: 7 in, 1 out]
                n171 = case shown="No Error" w473 {
                  tunnel: w472 -> [w480 _]
                  tunnel: w471 -> [w479 w494]
                  tunnel: [w478 w494] -> w470
                  tunnel: w469 -> [w477 w493]
                  tunnel: [w476 w493] -> w468
                  tunnel: w467 -> [w475 _]
                  tunnel: w465 -> [w474 _]
                  frame No Error {
                    n172 = case shown="-1" w474 {
                      tunnel: w480 -> [w486 w492]
                      tunnel: w479 -> [w485 w491]
                      tunnel: [w484 w490] -> w478
                      tunnel: w477 -> [w483 w489]
                      tunnel: [w482 w488] -> w476
                      tunnel: w475 -> [w481 w487]
                      frame -1 {
                        n173 = Build Array (concatenate)(w483, w481) -> (w482:path[])
                        n174 = Build Array (concatenate)(w485, w486) -> (w484:refnum<vi>[])
                      }
                      frame Default {
                        n175 = Build Array (concatenate)(w487, w489) -> (w488:path[])
                        n176 = Build Array (concatenate)(w492, w491) -> (w490:refnum<vi>[])
                      }
                    }
                  }
                  frame Error {
                  }
                }
              }
            }
          }
          n177 = Bundle By Name(cluster=w435, "ViRefs"=w434, "ViPathes"=w431) -> (w433:T2)
        }
        n178 = property on="Progress" class="LstBox (strict)"() -> ("Item Names"=w420:string[])  [unwired: 2 in, 2 out]
        n179 = Build Array (concatenate)(w420, "Loading Class VIs in memory") -> (w419:string[])
        n180 = Bundle By Name(cluster=w426, "Classes"=w422) -> (w425:T7)
        n181 = property on="Progress" class="LstBox (strict)"("Item Names"=w419) -> ()  [unwired: 2 in, 2 out]
      }
      frame "AnalyseClass" {
        n182 = Unbundle By Name(w503) -> ("AppRef"=w501:refnum<vi>, "Classes"=w497:T2[])
        n183 = for {
          tunnel: w497 -> [w509] mode=indexing
          tunnel: [w506] -> w496 mode=indexing
          tunnel: [w505] -> w495 mode=indexing
          n184 = Unbundle By Name(w509) -> ("ClassFolder"=w506:path, "ClassName"=w507:string)
          n185 = Concatenate Strings(w507, ".lvclass" ("string")) -> (w505:string)
        }
        n186 = for {
          tunnel: w497 -> [w519] mode=indexing
          tunnel: [w518] -> w498 mode=indexing
          tunnel: w501 -> [w516]
          tunnel: w496 -> [w512]
          tunnel: w495 -> [w511]
          n187 = Unbundle By Name(w519) -> ("ClassFolder"=w524:path)
          n188 = call <vilib>:"Recursive File List.vi"("pattern"="*GoopKernel.vi", "Treat LLBs as Folders?"=TRUE, "Folder Path"=w524) -> ("All Files in Dir"=w522:path[])  [unwired: 4 in, 4 out]
          n189 = Index Array(array=w522) -> (element=w521:path)  [unwired: 1 in]
          n190 = call "ConvertGoop2ToGoop3_GetGoop2ClassInheritance.vi"("application reference (local)"=w516, "Goop2VIPath(has to use GOOPKernel)"=w521) -> ("Inheritance"=w513:path[])  [unwired: 16 in, 1 out]
          n191 = Index Array(array=w513) -> (element=w517:path)  [unwired: 1 in]
          n192 = Delete From Array(array=w513) -> (deleted portion=w515:path)  [unwired: 2 in, 1 out]
          n193 = for {
            tunnel: w513 -> [w528] mode=indexing
            tunnel: w512 -> [w529]
            tunnel: w511 -> [w527]
            tunnel: [w525] -> w510 mode=indexing
            n194 = Search 1D Array(1D array=w529, element=w528) -> (index of element=w526:i32)  [unwired: 1 in]
            n195 = Index Array(array=w527, index=w526) -> (element=w525:string)
          }
          n196 = Array Size(array=w513) -> (size(s)=w514:i32)
          n197 = Bundle By Name(cluster=w519, "NoOfInheritance"=w514, "InheritsFrom"=w517, "RootClass"=w515, "AllInheritanceClasses"=w510) -> (w518:T2)
        }
        n198 = Sort 1D Array(array=w498) -> (sorted array=w499:T2[])
        n199 = Bundle By Name(cluster=w503, "Classes"=w499) -> (w502:T7)
      }
      frame "RemoveReentrantForDynamicDispatchVIs" {
        n200 = Unbundle By Name(w534) -> ("Classes"=w531:T2[])
        n201 = for {
          tunnel: w531 -> [w544] mode=indexing
          shift-right: [w542] -> w532
          shift-left: w533 -> [w543]
          tunnel: w531 -> [w539]
          i -> [w538]
          n202 = Delete From Array(array=w539, index=w538) -> (array with subset deleted=w537:T2[])  [unwired: 1 in, 1 out]
          n203 = Unbundle By Name(w544) -> ("ViRefs"=w541:refnum<vi>[], "ViPathes"=w540:path[])
          n204 = for {
            tunnel: w537 -> [w549] mode=indexing
            shift-right: [w547] -> w535
            shift-left: string[] [] -> [w548]
            n205 = Unbundle By Name(w549) -> ("ViPathes"=w545:path[])
            n206 = for {
              tunnel: [w551] -> w546 mode=indexing
              tunnel: w545 -> [w550] mode=indexing
              n207 = Strip Path(path=w550) -> (name=w551:string)  [unwired: 1 out]
            }
            n208 = Build Array (concatenate)(w548, w546) -> (w547:string[])
          }
          n209 = for {
            shift-right: [w564] -> w542
            shift-left: w543 -> [w565]
            tunnel: w541 -> [w563] mode=indexing
            tunnel: w540 -> [w562] mode=indexing
            tunnel: w535 -> [w555]
            n210 = Strip Path(path=w562) -> (stripped path=w561:path, name=w557:string)
            n211 = To Lower Case(string=w555) -> (all lower case string=w554:string[])
            n212 = To Lower Case(string=w557) -> (all lower case string=w556:string)
            n213 = Strip Path(path=w561) -> (name=w560:string)  [unwired: 1 out]
            n214 = Search 1D Array(1D array=w554, element=w556) -> (index of element=w553:i32)  [unwired: 1 in]
            n215 = Not Equal?(x=w560, y="utils") -> (x != y?=w558:bool)
            n216 = Greater Or Equal To 0?(x=w553) -> (x >= 0?=w552:bool)
            n217 = case shown="True" w558 {
              tunnel: w565 -> [w566 w567]
              tunnel: [w566 w567] -> w564
              tunnel: w563 -> [_ w569]
              tunnel: w552 -> [_ _]
              frame False {
              }
              frame True {
                n218 = property class="VI"(reference=w569, error in=w567, "Exec.IsReentrant"=FALSE ("Execution:Is Reentrant")) -> ()  [unwired: 2 out]
              }
            }
          }
        }
      }
      frame "RecompilingVIs" {
        n219 = call "ConvertGoop2ToGoop3_RecompileAll.vi"("error IO 2"=w576, "Cluster 2"=w575) -> ("error IO"=w574:errorcluster)  [unwired: 7 in]
        n220 = property on="Progress" class="LstBox (strict)"() -> ("Item Names"=w572:string[])  [unwired: 2 in, 2 out]
        n221 = Build Array (concatenate)(w572, "Recompiling VIs") -> (w571:string[])
        n222 = property on="Progress" class="LstBox (strict)"("Item Names"=w571) -> ()  [unwired: 2 in, 2 out]
      }
      frame "AddVIsToProject" {
        n223 = Unbundle By Name(w579) -> ("ProjectRef"=w578:refnum<vi>, "My Computer"=w577:refnum<vi>)
        n224 = Unbundle By Name(w579) -> ("TopFolderPath"=w580:path, "VIsToRelink(Paths)"=w587:path[])
        n225 = for {
          tunnel: w587 -> [w589] mode=indexing
          shift-right: [w588] -> w582
          shift-left: w586 -> [w588]
          tunnel: w580 -> [w596]
          tunnel: w577 -> [w592]
          tunnel: w578 -> [w591]
          n226 = Strip Path(path=w589) -> (stripped path=w595:path, name=w590:string)
          n227 = call <vilib>:"Compare Two Paths.vi"("Path 2"=w595, "Path 1"=w596) -> ("Relative Path from 1 to 2"=w594:path)  [unwired: 6 in, 3 out]
          n228 = Path To String(path=w594) -> (string=w593:string)
          n229 = case shown="Default" w593 {
            selector: w593 -> [w610 _]
            tunnel: w592 -> [w609 w614]
            tunnel: w591 -> [w599 _]
            tunnel: w588 -> [w606 _]
            tunnel: w590 -> [w605 w615]
            tunnel: w589 -> [w604 w616]
            tunnel: [w600 w613] -> _
            frame Default {
              n230 = call "GDSProject_CreateFolder.vi"("Project Refnum In"=w599, "Project Item To Create Folder Below(Use MyComputer if not wired)"=w609, "FolderName"=w610, "error in (no error)"=w606) -> ("ItemOut"=w598:refnum<vi>, "error out"=w607:errorcluster)  [unwired: 12 in, 2 out]
              n231 = invoke class="ProjectItem" method="AddItem"(reference=w598, error in=w607, "Name"=w605, "Path"=w604, "Type"="VI") -> (reference out=w602:refnum<vi>, error out=w603:errorcluster, "AddItem"=w597:refnum<vi>)  [unwired: 1 in, 3 out]
              n232 = Close Reference(reference=w602, error in (no error)=w603) -> (error out=w601:errorcluster)
              n233 = Close Reference(reference=w597, error in (no error)=w601) -> (error out=w600:errorcluster)
            }
            frame "", "." {
              n234 = invoke class="TargetItem" method="AddItem"(reference=w614, "Name"=w615, "Path"=w616, "Type"="VI") -> (error out=w611:errorcluster, "AddItem"=w612:refnum<vi>)  [unwired: 2 in, 4 out]
              n235 = Close Reference(reference=w612, error in (no error)=w611) -> (error out=w613:errorcluster)
            }
          }
        }
        n236 = property on="Progress" class="LstBox (strict)"() -> ("Item Names"=w585:string[])  [unwired: 2 in, 2 out]
        n237 = Build Array (concatenate)(w585, "Adding VIs to project") -> (w584:string[])
        n238 = property on="Progress" class="LstBox (strict)"("Item Names"=w584) -> ()  [unwired: 2 in, 2 out]
      }
      frame "RenameFiles" {
        n239 = Unbundle By Name(w619) -> ("My Computer"=w622:refnum<vi>, "TopFolderPath"=w627:path)
        n240 = Unbundle By Name(w619) -> ("Classes"=w628:T2[])
        n241 = for {
          tunnel: w628 -> [w651] mode=indexing
          tunnel: w627 -> [_]
          shift-right: [w637] -> w626
          shift-left: w625 -> [w630]
          tunnel: [w658] -> w623 mode=indexing
          tunnel: w622 -> [w636]
          shift-right: [w653] -> w621
          shift-left: path[] [] -> [w654]
          tunnel: w619 -> [w650]
          n242 = Unbundle By Name(w651) -> ("ClassName"=w633:string, "ClassFolder"=w655:path, "ClassPrefix"=w659:string, "ViRefs"=w652:refnum<vi>[])
          n243 = Unbundle By Name(w651) -> ("ClassName"=w656:string)
          n244 = Format Into String(format string="Renaming class: %s", w656) -> (resulting string=w641:string)  [unwired: 2 in, 1 out]
          n245 = property on="Progress" class="LstBox (strict)"() -> ("Item Names"=w649:string[], "Number of Rows"=w643:u32)  [unwired: 2 in, 2 out]
          n246 = Build Array (concatenate)(w649, w641) -> (w644:string[])
          n247 = Array Size(array=w644) -> (size(s)=w648:i32)
          n248 = Subtract(x=w648, y=w643) -> (x-y=w647:u32)
          n249 = To Long Integer(number=w647) -> (32bit integer=w645:i32)
          n250 = Max & Min(x=w645, y=0) -> (max(x,y)=w642:i32)  [unwired: 1 out]
          n251 = property on="Progress" class="LstBox (strict)"("Item Names"=w644, "Top Row"=w642) -> (error out=w640:errorcluster)  [unwired: 2 in, 1 out]
          n252 = for {
            tunnel: w652 -> [w685] mode=indexing
            shift-right: [w662] -> _
            shift-left: w630 -> [w662]
            tunnel: w659 -> [w683]
            tunnel: [w680] -> w638 mode=indexing
            tunnel: w655 -> [w679]
            tunnel: [w678] -> w632
            shift-right: [w676] -> w653
            shift-left: w654 -> [w675]
            tunnel: [w672] -> w634 mode=indexing
            tunnel: w650 -> [w669]
            tunnel: w640 -> [_]
            tunnel: [w663] -> _
            n253 = property class="VI"(reference=w685, error in=w662) -> (reference out=w684:refnum<vi>, error out=w671:errorcluster, "Path"=w677:path, "OwningApp"=w668:refnum<vi>)
            n254 = while {
              shift-right: [w686] -> w664
              shift-left: _ -> [w688]
              stop <- TRUE stop-if-true
              n255 = Increment(x=w688) -> (x+1=w687:i32)
              n256 = To Long Integer(number=w687) -> (32bit integer=w686:i32)
            }
            n257 = Strip Path(path=w677) -> ()  [unwired: 2 out]
            n258 = disable-structure shown="Disabled" {
              disable-tunnel: w671 -> [w693 w694]
              disable-tunnel: [w692 w694] -> w670
              disable-tunnel: w669 -> [w691 _]
              frame Disabled {
                n259 = call "ConvertGoop2ToGoop3_RecompileAll.vi"("error IO 2"=w693, "Cluster 2"=w691) -> ("error IO"=w692:errorcluster)  [unwired: 7 in]
              }
              frame Enabled {
              }
            }
            n260 = property class="App"(reference=w668) -> (reference out=w661:refnum<vi>, error out=w660:errorcluster, "App.Name"=w667:string)  [unwired: 1 in]
            n261 = Format Into String(format string="TempName%d.", w664) -> (resulting string=w665:string)  [unwired: 2 in, 1 out]
            n262 = call "ConvertGoop2ToGoop3_KeepViPrefix.vi"("OrgViName"=w677, "ClassFolder"=w679, "error in (no error)"=w670, "ClassPrefix"=w683) -> ("ClassFolderOut"=w678:path, "Don'tUseVI"=w673:bool, "NewClassPath"=w674:path, "NewClassPathWithPreFix"=w682:path, "error out"=w681:errorcluster)  [unwired: 10 in, 1 out]
            n263 = Close Reference(reference=w661, error in (no error)=w660) -> ()  [unwired: 1 out]
            n264 = case shown="False" w673 {
              tunnel: w684 -> [w714 w750]
              tunnel: w682 -> [w703 _]
              tunnel: w681 -> [w712 w747]
              tunnel: [w709 w745] -> w663
              tunnel: w674 -> [w700 _]
              tunnel: [w711 w746] -> w680
              tunnel: w677 -> [w708 w746]
              tunnel: w677 -> [_ w742]
              tunnel: [w707 w743] -> w676
              tunnel: w675 -> [w706 w744]
              tunnel: [w705 _] -> w672
              tunnel: w667 -> [w701 _]
              tunnel: w665 -> [w698 _]
              frame False {
                # "Remove\nPrefix ?"
                n265 = call <vilib>:"Get File Extension.vi"("file"=w700) -> ("filename without extension"=w699:string, "lowercase file extension"=w697:string)  [unwired: 6 in, 3 out]
                n266 = Strip Path(path=w703) -> (name=w702:string)  [unwired: 1 out]
                n267 = invoke class="VI" method="Save.Instrument"(reference=w714, error in=w712, "Path to saved file"=w700) -> (reference out=w705:refnum<vi>, error out=w713:errorcluster)  [unwired: 3 in, 4 out]
                n268 = Strip Path(path=w700) -> (stripped path=w696:path, name=w704:string)
                n269 = Concatenate Strings(w699, w698, w697) -> (w695:string)
                n270 = case shown="Error" w713 {
                  selector: w713 -> [w720 _]
                  tunnel: [w720 w727] -> w709
                  tunnel: w703 -> [_ w728]
                  tunnel: w712 -> [_ w730]
                  tunnel: w705 -> [_ w729]
                  tunnel: [w719 w728] -> w711
                  tunnel: w700 -> [w719 _]
                  tunnel: w704 -> [_ w726]
                  tunnel: w702 -> [_ w725]
                  tunnel: w701 -> [_ w724]
                  tunnel: w696 -> [_ w723]
                  tunnel: w695 -> [_ w722]
                  frame No Error {
                    # "Prefix\nRemoved"
                  }
                  frame Error {
                    # "..not\npossible"
                    n271 = Build Path(base path=w723, name or relative path=w722) -> (appended path=w721:path)
                    n272 = stacked-sequence {
                      tunnel: w726 -> [w733]
                      tunnel: w725 -> [w732]
                      tunnel: [w732] -> _
                      tunnel: w724 -> [w731]
                      frame #0 {
                        w737 = path "c:/G2To3.txt" ("file (use dialog)")
                        n273 = Read from Text File(file (use dialog)=w737) -> (text=w734:string)  [unwired: 3 in, 3 out]
                        n274 = Format Into String(format string="       %s(%s)%s\n", initial string=w734, w733, w732, w731) -> (resulting string=w736:string)  [unwired: 1 in, 1 out]
                        n275 = stacked-sequence {
                          tunnel: w736 -> [w740]
                          tunnel: w737 -> [w738]
                          frame #0 {
                            n276 = Delete(path (use dialog)=w738) -> (deleted path=w739:path)  [unwired: 4 in, 2 out]
                            n277 = Write to Text File(file (use dialog)=w739, text=w740) -> ()  [unwired: 2 in, 3 out]
                          }
                        }
                      }
                    }
                    n278 = invoke class="VI" method="Save.Instrument"(reference=w729, error in=w730, "Path to saved file"=w721) -> (error out=w727:errorcluster)  [unwired: 3 in, 5 out]
                  }
                }
                n279 = Not Equal?(x=w711, y=w708) -> (x != y?=w710:bool)
                n280 = case shown="False" w710 {
                  tunnel: w709 -> [_ _]
                  tunnel: w708 -> [_ w716]
                  tunnel: [w715 w718] -> w707
                  tunnel: w706 -> [w715 w717]
                  frame False {
                  }
                  frame True {
                    n281 = Build Array (concatenate)(w717, w716) -> (w718:path[])
                  }
                }
              }
              frame True {
                n282 = case shown="False" FALSE {
                  tunnel: w750 -> [w752 w756]
                  tunnel: [w752 w755] -> w749
                  tunnel: [w751 w754] -> w748
                  tunnel: w747 -> [w751 w753]
                  frame False {
                  }
                  frame True {
                    n283 = invoke class="VI" method="Save.Instrument"(reference=w756, error in=w753) -> (reference out=w755:refnum<vi>, error out=w754:errorcluster)  [unwired: 4 in, 4 out]
                  }
                }
                n284 = Close Reference(reference=w749, error in (no error)=w748) -> (error out=w745:errorcluster)
                n285 = Build Array (concatenate)(w744, w742) -> (w743:path[])
              }
            }
            n286 = stacked-sequence {
              tunnel: w663 -> [_]
              frame #0 {
                n287 = Wait (ms)(milliseconds to wait=u32 2) -> ()  [unwired: 1 out]
              }
            }
          }
          n288 = call "ConvertGoop2ToGoop3_CreateLvClass.vi"("ClassFolder"=w632, "ProjectItem"=w636, "ClassName"=w633, "ViRefsIn"=w634, "ViPathsIn"=w638, "error in"=w630) -> ("LvClassCreated"=w631:refnum<vi>, "ViRefsOut"=w635:refnum<vi>[], "ViPathsOut"=w639:path[], "error out"=w637:errorcluster)  [unwired: 6 in]
          n289 = Bundle By Name(cluster=w651, "ClassFolder"=w632, "ViRefs"=w635, "ViPathes"=w639, "ClassRef"=w631) -> (w658:T2)
        }
        n290 = Bundle By Name(cluster=w619, "Classes"=w623) -> (w624:T7)
        n291 = for {
          tunnel: w621 -> [w629] mode=indexing
          n292 = Delete(path (use dialog)=w629) -> ()  [unwired: 4 in, 3 out]
        }
      }
      frame "RenameTempNames" {
        n293 = Unbundle By Name(w758) -> ("Classes"=w761:T2[])
        n294 = for {
          tunnel: w761 -> [w763] mode=indexing
          shift-right: [w762] -> w760
          shift-left: w757 -> [w766]
          tunnel: w758 -> [w764]
          n295 = Unbundle By Name(w763) -> ("ViRefs"=w765:refnum<vi>[])
          n296 = for {
            tunnel: w765 -> [w772] mode=indexing
            shift-right: [w769] -> w762
            shift-left: w766 -> [w767]
            tunnel: w764 -> [_]
            n297 = property class="VI"(reference=w772, error in=w767) -> (reference out=w770:refnum<vi>, error out=w768:errorcluster, "Path"=w771:path)
            n298 = case shown="No Error" w768 {
              selector: w768 -> [w773 _]
              tunnel: w771 -> [w777 _]
              tunnel: w770 -> [w776 _]
              tunnel: [w775 w792] -> w769
              tunnel: w767 -> [_ w792]
              frame No Error {
                n299 = call <vilib>:"Get File Extension.vi"("file"=w777) -> ("filename without extension"=w781:string)  [unwired: 6 in, 4 out]
                n300 = Match Pattern(string=w781, regular expression="TempName[0-9]+") -> (before substring=w779:string, after substring=w778:string, offset past match=w774:i32)  [unwired: 1 in, 1 out]
                n301 = case shown="0, Default" w774 {
                  tunnel: w779 -> [w790 _]
                  tunnel: w778 -> [w789 _]
                  tunnel: w777 -> [w788 _]
                  tunnel: w776 -> [w785 _]
                  tunnel: w773 -> [w784 w791]
                  tunnel: [w783 w791] -> w775
                  frame 0, Default {
                    n302 = Concatenate Strings(w790, w789) -> (w786:string)
                    n303 = Strip Path(path=w788) -> (stripped path=w787:path)  [unwired: 1 out]
                    n304 = Build Path(base path=w787, name or relative path=w786) -> (appended path=w782:path)
                    n305 = invoke class="VI" method="Save.Instrument"(reference=w785, error in=w784, "Path to saved file"=w782) -> (error out=w783:errorcluster)  [unwired: 3 in, 5 out]
                  }
                  frame -1 {
                  }
                }
              }
              frame Error {
              }
            }
          }
        }
      }
      frame "FindAllCallParentMethodCalls" {
        n306 = Unbundle By Name(w797) -> ("Classes"=w800:T2[])
        n307 = for {
          tunnel: w800 -> [w807] mode=indexing
          shift-right: [w805] -> w798
          shift-left: w799 -> [w818]
          shift-right: [w801] -> w795
          shift-left: cluster{"VI Refnum":refnum<vi>, "Position":T6}[] [] -> [w802]
          n308 = Unbundle By Name(w807) -> ("ClassName"=w806:string)
          n309 = Unbundle By Name(w807) -> ("ViRefs"=w804:refnum<vi>[], "AllInheritanceClasses"=w803:string[])
          n310 = for {
            shift-right: [w824] -> w805
            shift-left: w818 -> [w826]
            tunnel: w803 -> [w825]
            tunnel: w804 -> [w821] mode=indexing
            shift-right: [w822] -> w801
            shift-left: w802 -> [w823]
            # "Does this VI call a Parent Method VI with te same name,\nIf so It shoule be peplaced by a CallParentMethod-function"
            n311 = Not A Number/Path/Refnum?(number/path/refnum=w821) -> (NaN/Path/Refnum?=w820:bool)
            n312 = case shown="False" w820 {
              tunnel: w826 -> [w842 w880]
              tunnel: w825 -> [w841 _]
              tunnel: [w832 w880] -> w824
              tunnel: w823 -> [w830 w879]
              tunnel: [w829 w879] -> w822
              tunnel: w821 -> [w828 _]
              frame False {
                n313 = property class="VI"(reference=w828, error in=w842) -> (reference out=w831:refnum<vi>, error out=w833:errorcluster, "VIType"=w834:T13, "Callees"=w839:string[], "Name"=w837:string)
                n314 = Match Pattern(string=w837, regular expression=":") -> (after substring=w835:string)  [unwired: 1 in, 3 out]
                n315 = for {
                  tunnel: w841 -> [w878] mode=indexing
                  tunnel: w835 -> [w877]
                  tunnel: [w875] -> w827 mode=indexing
                  n316 = Concatenate Strings(w878, ":" ("string"), w877) -> (w875:string)
                }
                n317 = To Lower Case(string=w839) -> (all lower case string=w838:string[])
                n318 = To Lower Case(string=w827) -> (all lower case string=w840:string[])
                n319 = case shown="\"Standard VI\"" w834 {
                  tunnel: w840 -> [_ w854]
                  tunnel: w838 -> [_ w853]
                  tunnel: w833 -> [w844 w850]
                  tunnel: [w844 w849] -> w832
                  tunnel: w827 -> [_ w845]
                  tunnel: w831 -> [_ w848]
                  tunnel: w830 -> [w843 w847]
                  tunnel: [w843 w846] -> w829
                  frame Default {
                  }
                  frame "Standard VI" {
                    n320 = for {
                      tunnel: w854 -> [w873] mode=indexing
                      tunnel: w853 -> [w874]
                      tunnel: [w871] -> w852 mode=indexing
                      n321 = Search 1D Array(1D array=w874, element=w873) -> (index of element=w872:i32)  [unwired: 1 in]
                      n322 = Greater Or Equal To 0?(x=w872) -> (x >= 0?=w871:bool)
                    }
                    n323 = Or Array Elements(Boolean array=w852) -> (logical OR=w851:bool)
                    n324 = case shown="True" w851 {
                      tunnel: w850 -> [w855 w863]
                      tunnel: [w855 w862] -> w849
                      tunnel: w845 -> [_ w861]
                      tunnel: w848 -> [_ w858]
                      tunnel: w847 -> [w856 w859]
                      tunnel: [w856 w857] -> w846
                      frame False {
                      }
                      frame True {
                        n325 = call "Scripting_FindVisOnDiagram.vi"("ViRef"=w858, "VIsToSerachFor/ViName"=w861, "error in (no error)"=w863) -> ("VisFound"=w860:refnum<vi>[], "error out"=w862:errorcluster)  [unwired: 15 in]
                        n326 = for {
                          tunnel: w860 -> [w870] mode=indexing
                          shift-right: [w865] -> w857
                          shift-left: w859 -> [w867]
                          tunnel: w858 -> [w868]
                          n327 = property class="GObj"(reference=w870) -> (reference out=w864:refnum<vi>, "Position"=w869:T6)  [unwired: 1 in, 1 out]
                          n328 = Bundle("VI Refnum"=w868, "Position"=w869) -> (w866:cluster{"VI Refnum":refnum<vi>, "Position":T6})  [unwired: 1 in]
                          n329 = Build Array (concatenate)(w867, w866) -> (w865:cluster{"VI Refnum":refnum<vi>, "Position":T6}[])
                          n330 = Close Reference(reference=w864) -> ()  [unwired: 1 in, 1 out]
                        }
                      }
                    }
                  }
                }
              }
              frame True {
              }
            }
          }
          n331 = Format Into String(format string="Searching Call Parent Method: %s", w806) -> (resulting string=w809:string)  [unwired: 2 in, 1 out]
          n332 = property on="Progress" class="LstBox (strict)"() -> ("Item Names"=w817:string[], "Number of Rows"=w811:u32)  [unwired: 2 in, 2 out]
          n333 = Build Array (concatenate)(w817, w809) -> (w812:string[])
          n334 = Array Size(array=w812) -> (size(s)=w816:i32)
          n335 = Subtract(x=w816, y=w811) -> (x-y=w815:u32)
          n336 = To Long Integer(number=w815) -> (32bit integer=w813:i32)
          n337 = Max & Min(x=w813, y=0) -> (max(x,y)=w810:i32)  [unwired: 1 out]
          n338 = property on="Progress" class="LstBox (strict)"("Item Names"=w812, "Top Row"=w810) -> ()  [unwired: 2 in, 2 out]
          n339 = stacked-sequence {
            tunnel: w805 -> [_]
            frame #0 {
              n340 = Wait (ms)(milliseconds to wait=u32 5) -> ()  [unwired: 1 out]
            }
          }
        }
        n341 = Bundle By Name(cluster=w797, "CallParentMethod"=w795) -> (w796:T7)
      }
      frame "UpdateNewVI" {
        n342 = Unbundle By Name(w881) -> ("Classes"=w895:T2[])
        n343 = call "ConvertGoop2ToGoop3_RecompileAll.vi"("error IO 2"=w883, "Cluster 2"=w881) -> ("error IO"=w882:errorcluster)  [unwired: 7 in]
        n344 = for {
          tunnel: w895 -> [w906] mode=indexing
          shift-right: [w904] -> w894
          shift-left: w882 -> [w905]
          n345 = Unbundle By Name(w906) -> ("ViRefs"=w903:refnum<vi>[], "ClassFolder"=w902:path, "ClassName"=w901:string)
          n346 = Concatenate Strings(w901, "_New.vi" ("string")) -> (w897:string)
          n347 = Build Path(base path=w902, name or relative path="Utils") -> (appended path=w899:path)
          n348 = Build Path(base path=w899, name or relative path=w897) -> (appended path=w896:path)
          n349 = for {
            tunnel: w903 -> [w912] mode=indexing
            shift-right: [w907] -> w904
            shift-left: w905 -> [w917]
            tunnel: w896 -> [w913]
            n350 = property class="VI"(reference=w912) -> ("Name"=w911:string)  [unwired: 1 in, 2 out]
            n351 = Match Pattern(string=w911, regular expression="_Create\\2Evi$") -> (offset past match=w909:i32)  [unwired: 1 in, 3 out]
            n352 = call "Scripting_ConnecorPaneRewiring.vi"("ViRef"=w912, "SubViThatHasChangedConnectorPane"=w913, "OldConnectorPaneIndex"=u32[] [6], "NewConnectorPaneIndex"=u32[] [8], "error in (no error)"=w917) -> ("error out"=w914:errorcluster)  [unwired: 14 in]
            n353 = case shown="-1" w909 {
              tunnel: w914 -> [w918 w923]
              tunnel: [w918 w922] -> w908
              tunnel: w913 -> [_ w920]
              tunnel: w912 -> [_ w919]
              frame 0, Default {
              }
              frame -1 {
                n354 = call "Scripting_ConnecorPaneCreateConstant.vi"("ViRef"=w919, "SubViThatHasChangedConnectorPane"=w920, "ConnectorPaneIndexToCReateConstantsOn"=u32[] [6, 0] ("OldConnectorPaneIndex"), "error in (no error)"=w923) -> ("error out"=w922:errorcluster)  [unwired: 15 in]
              }
            }
            n355 = call <vilib>:"Clear Errors.vi"("error in (no error)"=w908) -> ("error out"=w907:errorcluster)  [unwired: 5 in, 1 out]
            n356 = stacked-sequence {
              tunnel: w907 -> [_]
              frame #0 {
                n357 = Wait (ms)(milliseconds to wait=u32 2) -> ()  [unwired: 1 out]
              }
            }
          }
        }
        n358 = property on="Progress" class="LstBox (strict)"() -> ("Item Names"=w892:string[], "Number of Rows"=w886:u32)  [unwired: 2 in, 2 out]
        n359 = Build Array (concatenate)(w892, "Update NEW-VI (due to cone-pane changes)") -> (w887:string[])
        n360 = Array Size(array=w887) -> (size(s)=w891:i32)
        n361 = Subtract(x=w891, y=w886) -> (x-y=w890:u32)
        n362 = To Long Integer(number=w890) -> (32bit integer=w888:i32)
        n363 = Max & Min(x=w888, y=0) -> (max(x,y)=w885:i32)  [unwired: 1 out]
        n364 = property on="Progress" class="LstBox (strict)"("Item Names"=w887, "Top Row"=w885) -> ()  [unwired: 2 in, 2 out]
      }
      frame "SetInheritance" {
        n365 = Unbundle By Name(w930) -> ("Classes"=w928:T2[])
        n366 = for {
          tunnel: w928 -> [w934] mode=indexing
          tunnel: [w933] -> w927 mode=indexing
          tunnel: [w932] -> w926 mode=indexing
          n367 = Unbundle By Name(w934) -> ("ClassName"=w933:string, "ClassRef"=w932:refnum<vi>)
        }
        n368 = for {
          tunnel: w928 -> [w950] mode=indexing
          shift-right: [w935] -> w931
          shift-left: w929 -> [w945]
          tunnel: w927 -> [w947]
          tunnel: w926 -> [w946]
          n369 = Unbundle By Name(w950) -> ("ClassName"=w940:string, "ClassRef"=w949:refnum<vi>, "InheritsFrom"=w948:path)
          n370 = Strip Path(path=w948) -> (name=w943:string)  [unwired: 1 out]
          n371 = Match Pattern(string=w943, regular expression="_[Cc][Ll][Aa][Ss][Ss]") -> (before substring=w938:string)  [unwired: 1 in, 3 out]
          n372 = Match Pattern(string=w938, regular expression="[.][Ll][Ll][Bb]$") -> (before substring=w936:string)  [unwired: 1 in, 3 out]
          n373 = Format Into String(format string="Setting inheritance: %s->%s", w940, w936) -> (resulting string=w939:string)  [unwired: 2 in, 1 out]
          n374 = Search 1D Array(1D array=w947, element=w936) -> (index of element=w944:i32)  [unwired: 1 in]
          n375 = case shown="0, Default" w944 {
            tunnel: w949 -> [w968 _]
            tunnel: w944 -> [w967 _]
            tunnel: w946 -> [w966 _]
            tunnel: w945 -> [w964 w969]
            tunnel: [w961 w969] -> w935
            tunnel: w939 -> [w952 _]
            frame 0, Default {
              n376 = Index Array(array=w966, index=w967) -> (element=w965:refnum<vi>)
              n377 = property class="LVClassLibrary"(reference=w968, error in=w964, "Parent"=w965) -> (reference out=w963:refnum<vi>, error out=w962:errorcluster)
              n378 = property on="Progress" class="LstBox (strict)"() -> ("Item Names"=w960:string[], "Number of Rows"=w954:u32)  [unwired: 2 in, 2 out]
              n379 = Build Array (concatenate)(w960, w952) -> (w955:string[])
              n380 = Array Size(array=w955) -> (size(s)=w959:i32)
              n381 = Subtract(x=w959, y=w954) -> (x-y=w958:u32)
              n382 = To Long Integer(number=w958) -> (32bit integer=w956:i32)
              n383 = Max & Min(x=w956, y=0) -> (max(x,y)=w953:i32)  [unwired: 1 out]
              n384 = invoke class="LVClassLibrary" method="Save"(reference=w963, error in=w962) -> (error out=w961:errorcluster)  [unwired: 2 in, 3 out]
              n385 = property on="Progress" class="LstBox (strict)"("Item Names"=w955, "Top Row"=w953) -> ()  [unwired: 2 in, 2 out]
            }
            frame -1 {
            }
          }
          n386 = stacked-sequence {
            tunnel: w935 -> [_]
            frame #0 {
              n387 = Wait (ms)(milliseconds to wait=u32 2) -> ()  [unwired: 1 out]
            }
          }
        }
      }
      frame "UpdateLvClassIcon" {
        n388 = Unbundle By Name(w984) -> ("Classes"=w983:T2[], "AppRef"=w979:refnum<vi>)
        n389 = for {
          tunnel: w983 -> [w1027] mode=indexing
          shift-right: [w986] -> w982
          shift-left: w981 -> [w1001]
          tunnel: w979 -> [w993]
          n390 = Unbundle By Name(w1027) -> ("ClassRef"=w994:refnum<vi>, "ClassFolder"=w1016:path)
          n391 = List Folder(path=w1016, pattern="*.vi") -> (filenames=w1018:string[])  [unwired: 2 in, 3 out]
          n392 = Index Array(array=w1018) -> (element=w1017:string)  [unwired: 1 in]
          n393 = Build Path(base path=w1016, name or relative path=w1017) -> (appended path=w1000:path)
          n394 = call "Scripting_OpenViRef.vi"("error in"=w1001, "ViPath/ViName/Viref"=w1000, "AppRef"=w993) -> ("error out"=w1002:errorcluster, "vi reference"=w998:refnum<vi>)  [unwired: 6 in, 1 out]
          n395 = call "GDSLvIcon_AnalyseViIcon.vi"("ViRef/LvCLassRef/LvLibRef/ViPath/2D_Image"=w998, "error in (no error)"=w1002) -> ("FrameColor"=w1015:u32, "FrameThickness(1)"=w1013:u32, "HeaderIcon"=w1008:u8[][], "HeaderBkColor"=w1003:u32, "BodyBkColor"=w1014:u32, "error out"=w999:errorcluster)  [unwired: 5 in, 7 out]
          n396 = Array Size(array=w1008) -> (size(s)=w1007:i32[])
          n397 = Close Reference(reference=w998, error in (no error)=w999) -> ()  [unwired: 1 out]
          n398 = Index Array(array=w1007) -> (element=w1005:i32)  [unwired: 1 in]
          n399 = Subtract(x=u32 32 ("Width(30)"), y=w1005) -> (x-y=w1004:u32)
          n400 = Multiply(x=w1013, y=u32 2) -> (x*y=w1011:u32)
          n401 = Subtract(x=u32 32 ("Width(30)"), y=w1011) -> (x-y=w1009:u32)
          n402 = call "GDSLvIcon_GenerateObjectIcon.vi"("HeaderColor"=w1003, "BackgroundColor"=w1014, "Height"=w1004, "error in (no error)"=w999, "Type"=enum16{"LvClass", "Library", "X-Control"}."LvClass", "Width(30)"=w1009) -> ("BodyIconOut"=w1020:u8[][], "error out"=w1021:errorcluster)  [unwired: 12 in]
          n403 = call "GDSLvIcon_CreateIconPicture.vi"("FrameColor"=w1015, "FrameThickness(1)"=w1013, "HeaderIconIn"=w1008, "BodyIconIn"=w1020, "error in (no error)"=w1021) -> ("WholeIconOut"=w1025:u8[][], "error out"=w1022:errorcluster)  [unwired: 9 in, 4 out]
          n404 = Reshape Array(w1025, 1024 ("dimension size")) -> (w1023:u8[])
          n405 = Bundle By Name(cluster=T9 {"image type"=0, "image depth"=8, "image"=[], "mask"=[], "colors"=[], "Rectangle"={"left"=0, "top"=0, "right"=32, "bottom"=32}} ("image data"), "image"=w1023) -> (w996:T9)
          n406 = invoke class="LVClassLibrary" method="Set Icon"(reference=w994, error in=w1022, "color"=w996) -> (reference out=w989:refnum<vi>, error out=w990:errorcluster)  [unwired: 2 in, 3 out]
          n407 = property class="LVClassLibrary"(reference=w989, error in=w990) -> (reference out=w988:refnum<vi>, error out=w995:errorcluster, "Member Data"=w997:refnum<vi>)
          n408 = invoke class="VI" method="VI Icon.Set from Image Data"(reference=w997, error in=w995, "ImageData"=w996) -> (reference out=w991:refnum<vi>, error out=w992:errorcluster)  [unwired: 3 in, 4 out]
          n409 = Close Reference(reference=w991, error in (no error)=w992) -> (error out=w987:errorcluster)
          n410 = invoke class="LVClassLibrary" method="Save"(reference=w988, error in=w987) -> (error out=w986:errorcluster)  [unwired: 2 in, 3 out]
          n411 = stacked-sequence {
            tunnel: w986 -> [_]
            frame #0 {
              n412 = Wait (ms)(milliseconds to wait=u32 2) -> ()  [unwired: 1 out]
            }
          }
        }
        n413 = property on="Progress" class="LstBox (strict)"() -> ("Item Names"=w978:string[], "Number of Rows"=w972:u32)  [unwired: 2 in, 2 out]
        n414 = Build Array (concatenate)(w978, string[] ["Updating Icons"] ("element")) -> (w973:string[])
        n415 = Array Size(array=w973) -> (size(s)=w977:i32)
        n416 = Subtract(x=w977, y=w972) -> (x-y=w976:u32)
        n417 = To Long Integer(number=w976) -> (32bit integer=w974:i32)
        n418 = Max & Min(x=w974, y=0) -> (max(x,y)=w971:i32)  [unwired: 1 out]
        n419 = property on="Progress" class="LstBox (strict)"("Item Names"=w973, "Top Row"=w971) -> ()  [unwired: 2 in, 2 out]
      }
      frame "UpdateLvClassAttributes" {
        n420 = Unbundle By Name(w1031) -> ("Classes"=w1033:T2[])
        n421 = for {
          tunnel: w1033 -> [w1050] mode=indexing
          shift-right: [w1048] -> w1032
          shift-left: w1030 -> [w1048]
          n422 = Unbundle By Name(w1050) -> ("ClassName"=w1035:string, "ClassRef"=w1049:refnum<vi>)
          n423 = call "Scripting_PlaceGoopRefInClassAttribute.vi"("error in"=w1048, "ClassRefnum"=w1049) -> ("error out"=w1047:errorcluster, "ClusterTypeDefPath"=w1045:path, "ObjectRef.ctl"=w1046:path)  [unwired: 2 in, 1 out]
          n424 = case shown="Error" w1047 {
            tunnel: w1035 -> [_ w1056]
            tunnel: w1046 -> [_ w1054]
            tunnel: w1045 -> [_ w1052]
            frame No Error {
              n425 = stacked-sequence {
                frame #0 {
                  n426 = Wait (ms)(milliseconds to wait=u32 2) -> ()  [unwired: 1 out]
                }
              }
            }
            frame Error {
              w1060 = path "c:/G2To3.txt" ("file (use dialog)")
              n427 = Path To String(path=w1052) -> (string=w1053:string)
              n428 = Path To String(path=w1054) -> (string=w1055:string)
              n429 = Read from Text File(file (use dialog)=w1060) -> (text=w1057:string)  [unwired: 3 in, 3 out]
              n430 = Format Into String(format string="       Error %s(%s)%s\n", initial string=w1057, w1056, w1053, w1055) -> (resulting string=w1059:string)  [unwired: 1 in, 1 out]
              n431 = stacked-sequence {
                tunnel: w1059 -> [w1063]
                tunnel: w1060 -> [w1061]
                frame #0 {
                  n432 = Delete(path (use dialog)=w1061) -> (deleted path=w1062:path)  [unwired: 4 in, 2 out]
                  n433 = Write to Text File(file (use dialog)=w1062, text=w1063) -> ()  [unwired: 2 in, 3 out]
                }
              }
              n434 = call <vilib>:"Beep.vi"() -> ()  [unwired: 12 in]
            }
          }
          n435 = Format Into String(format string="Updating LvClass Attribute: %s", w1035) -> (resulting string=w1034:string)  [unwired: 2 in, 1 out]
          n436 = property on="Progress" class="LstBox (strict)"() -> ("Item Names"=w1044:string[], "Number of Rows"=w1038:u32)  [unwired: 2 in, 2 out]
          n437 = Build Array (concatenate)(w1044, w1034) -> (w1039:string[])
          n438 = Array Size(array=w1039) -> (size(s)=w1043:i32)
          n439 = Subtract(x=w1043, y=w1038) -> (x-y=w1042:u32)
          n440 = To Long Integer(number=w1042) -> (32bit integer=w1040:i32)
          n441 = Max & Min(x=w1040, y=0) -> (max(x,y)=w1037:i32)  [unwired: 1 out]
          n442 = property on="Progress" class="LstBox (strict)"("Item Names"=w1039, "Top Row"=w1037) -> ()  [unwired: 2 in, 2 out]
        }
      }
      frame "UpdateUtilsVIs" {
        n443 = Unbundle By Name(w1064) -> ("Classes"=w1072:T2[])
        n444 = local read "State"() -> (w1069:string)
        n445 = for {
          tunnel: w1072 -> [w1075] mode=indexing
          shift-right: [w1093] -> w1066
          shift-left: w1071 -> [w1094]
          tunnel: w1069 -> [w1077]
          tunnel: [w1073] -> w1068 mode=indexing
          n446 = Unbundle By Name(w1075) -> ("InheritsFrom"=w1101:path, "ClassName"=w1087:string, "ViRefs"=w1092:refnum<vi>[], "ViPathes"=w1090:path[])
          n447 = Empty String/Path?(string/path=w1101) -> (empty?=w1100:bool)
          n448 = Select(t=EndevoTemplateNames."BaseTemplate" ("TemplateNames"), s=w1100, f=EndevoTemplateNames."SubTemplate" ("TemplateNames")) -> (s? t:f=w1097:T10)
          n449 = Format Into String(w1097) -> (resulting string=w1089:string)  [unwired: 3 in, 1 out]
          n450 = call "GOOP300_GetClassTemplatePath.vi"("ClassTemplateSubDirectory"=w1089) -> ("FolderPathOut"=w1095:path)  [unwired: 17 in, 1 out]
          n451 = Build Path(base path=w1095, name or relative path="utils") -> (appended path=w1091:path)
          n452 = for {
            shift-right: [w1113] -> w1093
            shift-left: w1094 -> [w1114]
            tunnel: w1092 -> [w1112] mode=indexing
            tunnel: w1091 -> [w1111]
            tunnel: w1090 -> [w1110] mode=indexing
            tunnel: w1089 -> [w1108]
            shift-right: [w1104] -> _
            shift-left: w1077 -> [w1105]
            shift-right: [w1103] -> w1074
            shift-left: "1.0.0" ("TemplateVersionUsed") -> [w1102]
            n453 = Strip Path(path=w1110) -> (stripped path=w1107:path, name=w1109:string)
            n454 = Strip Path(path=w1107) -> (name=w1106:string)  [unwired: 1 out]
            n455 = case shown="\"utils\"" w1106 {
              tunnel: w1114 -> [w1117 w1135]
              tunnel: [w1117 w1134] -> w1113
              tunnel: w1112 -> [_ w1133]
              tunnel: w1111 -> [_ w1132]
              tunnel: w1109 -> [_ w1123]
              tunnel: w1108 -> [_ w1130]
              tunnel: w1105 -> [w1116 w1126]
              tunnel: [w1116 w1124] -> w1104
              tunnel: [w1115 w1119] -> w1103
              tunnel: w1102 -> [w1115 w1118]
              frame Default {
              }
              frame "utils" {
                w1131 = "_" ("regular expression")
                n456 = Reverse String(1:w1123) -> (0:w1122:string)
                n457 = Match Pattern(string=w1122, regular expression=w1131) -> (before substring=w1121:string)  [unwired: 1 in, 3 out]
                n458 = Concatenate Strings(w1126, "." ("string")) -> (w1124:string)
                n459 = Reverse String(1:w1121) -> (0:w1120:string)
                n460 = local write "State"(w1124) -> ()
                n461 = Concatenate Strings(w1130, w1131, w1120) -> (w1129:string)
                n462 = Build Path(base path=w1132, name or relative path=w1129) -> (appended path=w1128:path)
                n463 = File/Directory Info(path=w1128) -> (size=w1127:i64)  [unwired: 1 in, 6 out]
                n464 = case shown="1.." w1127 {
                  tunnel: w1135 -> [w1137 w1140]
                  tunnel: [w1137 w1140] -> w1134
                  tunnel: w1133 -> [_ w1142]
                  tunnel: w1128 -> [_ w1141]
                  tunnel: [w1136 w1138] -> w1119
                  tunnel: w1118 -> [w1136 _]
                  frame 0, Default {
                  }
                  frame 1.. {
                    n465 = call "Scripting_UpdateViFromTemplate.vi"("ViRef"=w1142, "TemplateVI(Path or Ref)"=w1141, "error in (no error)"=w1140) -> ("TemplateVersionUsed"=w1138:string, "error out"=w1139:errorcluster)  [unwired: 15 in]
                    n466 = stacked-sequence {
                      tunnel: w1139 -> [_]
                      frame #0 {
                        n467 = Wait (ms)(milliseconds to wait=u32 5) -> ()  [unwired: 1 out]
                      }
                    }
                  }
                }
              }
            }
          }
          n468 = Format Into String(format string="Updating utils VIs: %s", w1087) -> (resulting string=w1078:string)  [unwired: 2 in, 1 out]
          n469 = property on="Progress" class="LstBox (strict)"() -> ("Item Names"=w1086:string[], "Number of Rows"=w1080:u32)  [unwired: 2 in, 2 out]
          n470 = Build Array (concatenate)(w1086, w1078) -> (w1081:string[])
          n471 = Array Size(array=w1081) -> (size(s)=w1085:i32)
          n472 = Subtract(x=w1085, y=w1080) -> (x-y=w1084:u32)
          n473 = To Long Integer(number=w1084) -> (32bit integer=w1082:i32)
          n474 = Max & Min(x=w1082, y=0) -> (max(x,y)=w1079:i32)  [unwired: 1 out]
          n475 = property on="Progress" class="LstBox (strict)"("Item Names"=w1081, "Top Row"=w1079) -> ()  [unwired: 2 in, 2 out]
          n476 = Bundle By Name(cluster=w1075, "TemplateVersionUsed"=w1074) -> (w1073:T2)
        }
        n477 = Bundle By Name(cluster=w1064, "Classes"=w1068) -> (w1067:T7)
        n478 = call "ConvertGoop2ToGoop3_RecompileAll.vi"("error IO 2"=w1066, "Cluster 2"=w1064) -> ("error IO"=w1065:errorcluster)  [unwired: 7 in]
      }
      frame "UpdateSubClassKernels" {
        n479 = Unbundle By Name(w1144) -> ("Classes"=w1157:T2[])
        n480 = for {
          tunnel: w1157 -> [w1161] mode=indexing
          tunnel: [w1160] -> w1156 mode=indexing
          tunnel: [w1159] -> w1148 mode=indexing
          n481 = Unbundle By Name(w1161) -> ("ClassName"=w1160:string, "ClassFolder"=w1159:path)
        }
        n482 = Format Into String(EndevoTemplateNames."BaseTemplate" ("TemplateNames")) -> (resulting string=w1152:string)  [unwired: 3 in, 1 out]
        n483 = call "GOOP300_GetClassTemplatePath.vi"("ClassTemplateSubDirectory"=w1152) -> ("FolderPathOut"=w1153:path)  [unwired: 17 in, 1 out]
        n484 = Build Path(base path=w1153, name or relative path="utils") -> (appended path=w1151:path)
        n485 = Build Path(base path=w1151, name or relative path="BaseTemplate_GOOPKernel.vi") -> (appended path=w1149:path)
        n486 = for {
          tunnel: w1157 -> [w1183] mode=indexing
          shift-right: [w1170] -> w1146
          shift-left: w1158 -> [w1171]
          tunnel: w1156 -> [w1169]
          tunnel: w1149 -> [w1168]
          tunnel: w1148 -> [w1167]
          n487 = Unbundle By Name(w1183) -> ("InheritsFrom"=w1172:path, "ClassName"=w1165:string, "ViRefs"=w1177:refnum<vi>[], "ViPathes"=w1181:path[])
          n488 = for {
            tunnel: w1181 -> [w1188] mode=indexing
            tunnel: "GOOPKernel.vi$" ("regular expression") -> [w1186]
            tunnel: [w1184] -> w1179 mode=indexing
            n489 = Strip Path(path=w1188) -> (name=w1187:string)  [unwired: 1 out]
            n490 = Match Pattern(string=w1187, regular expression=w1186) -> (offset past match=w1185:i32)  [unwired: 1 in, 3 out]
            n491 = Greater Or Equal To 0?(x=w1185) -> (x >= 0?=w1184:bool)
          }
          n492 = Strip Path(path=w1172) -> (name=w1173:string)  [unwired: 1 out]
          n493 = Match Pattern(string=w1173, regular expression="_[Cc][Ll][Aa][Ss][Ss]") -> (before substring=w1164:string)  [unwired: 1 in, 3 out]
          n494 = Empty String/Path?(string/path=w1172) -> (empty?=w1182:bool)
          n495 = Match Pattern(string=w1164, regular expression="[.][Ll][Ll][Bb]$") -> (before substring=w1162:string)  [unwired: 1 in, 3 out]
          n496 = Search 1D Array(1D array=w1179, element=TRUE) -> (index of element=w1176:i32)  [unwired: 1 in]
          n497 = Index Array(array=w1177, index=w1176) -> (element=w1175:refnum<vi>)
          n498 = Search 1D Array(1D array=w1169, element=w1162) -> (index of element=w1166:i32)  [unwired: 1 in]
          n499 = case shown="False" w1182 {
            tunnel: w1175 -> [w1209 _]
            tunnel: w1171 -> [w1189 w1211]
            tunnel: [w1189 w1211] -> w1170
            tunnel: w1168 -> [w1208 _]
            tunnel: w1167 -> [w1206 _]
            tunnel: w1166 -> [w1205 _]
            tunnel: w1165 -> [w1200 _]
            frame False {
              n500 = Index Array(array=w1206, index=w1205) -> (element=w1204:path)
              n501 = call <vilib>:"Recursive File List.vi"("pattern"="*GOOPKernel.vi", "Treat LLBs as Folders?"=TRUE, "Folder Path"=w1204) -> ("All Files in Dir"=w1201:path[])  [unwired: 4 in, 4 out]
              n502 = Build Array(w1208) -> (w1207:path[])
              n503 = Format Into String(format string="Updating kernel: %s", w1200) -> (resulting string=w1190:string)  [unwired: 2 in, 1 out]
              n504 = call "Scripting_ReplaceVisAndControls.vi"("ViRef"=w1209, "OldVIsAndControls"=w1207, "NewVIsAndControls"=w1201, "error in (no error)"=w1189) -> ()  [unwired: 14 in, 2 out]
              n505 = property on="Progress" class="LstBox (strict)"() -> ("Item Names"=w1198:string[], "Number of Rows"=w1192:u32)  [unwired: 2 in, 2 out]
              n506 = Build Array (concatenate)(w1198, w1190) -> (w1193:string[])
              n507 = stacked-sequence {
                tunnel: w1189 -> [_]
                frame #0 {
                  n508 = Wait (ms)(milliseconds to wait=u32 5) -> ()  [unwired: 1 out]
                }
              }
              n509 = Array Size(array=w1193) -> (size(s)=w1197:i32)
              n510 = Subtract(x=w1197, y=w1192) -> (x-y=w1196:u32)
              n511 = To Long Integer(number=w1196) -> (32bit integer=w1194:i32)
              n512 = Max & Min(x=w1194, y=0) -> (max(x,y)=w1191:i32)  [unwired: 1 out]
              n513 = property on="Progress" class="LstBox (strict)"("Item Names"=w1193, "Top Row"=w1191) -> ()  [unwired: 2 in, 2 out]
            }
            frame True {
            }
          }
        }
        n514 = call "ConvertGoop2ToGoop3_RecompileAll.vi"("error IO 2"=w1146, "Cluster 2"=w1144) -> ("error IO"=w1145:errorcluster)  [unwired: 7 in]
      }
      frame "UpdateVIsGoopRefs" {
        n515 = Unbundle By Name(w1212) -> ("Classes"=w1219:T2[])
        n516 = for {
          tunnel: w1219 -> [w1233] mode=indexing
          tunnel: [w1231] -> w1215 mode=indexing
          n517 = Unbundle By Name(w1233) -> ("ClassRef"=w1232:refnum<vi>)
          n518 = property class="LVClassLibrary"(reference=w1232) -> ("Path"=w1231:path)  [unwired: 1 in, 2 out]
        }
        n519 = for {
          tunnel: w1219 -> [w1250] mode=indexing
          shift-right: [w1234] -> w1217
          shift-left: w1220 -> [w1249]
          tunnel: w1215 -> [w1247]
          n520 = Unbundle By Name(w1250) -> ("ViRefs"=w1248:refnum<vi>[], "ViPathes"=w1246:path[], "ClassName"=w1236:string)  [unwired: 2 out]
          n521 = for {
            shift-right: [w1264] -> w1234
            shift-left: w1249 -> [w1265]
            tunnel: w1248 -> [w1255] mode=indexing
            tunnel: w1247 -> [w1263]
            tunnel: w1246 -> [w1257] mode=indexing
            tunnel: [w1256] -> _
            n522 = Strip Path(path=w1257) -> (stripped path=w1262:path, name=w1259:string)
            n523 = Path To String(path=w1257) -> (string=w1256:string)
            n524 = Match Pattern(string=w1259, regular expression="\\2E[Vv][Ii]$") -> ()  [unwired: 1 in, 4 out]
            n525 = Strip Path(path=w1262) -> (name=w1261:string)  [unwired: 1 out]
            n526 = Not Equal?(x=w1261, y="utils") -> (x != y?=w1254:bool)
            n527 = Not A Number/Path/Refnum?(number/path/refnum=w1255) -> (NaN/Path/Refnum?=w1253:bool)
            n528 = Compound Arithmetic op=AND(invert w1253, w1254) -> (w1252:bool)
            n529 = case shown="True" w1252 {
              tunnel: w1265 -> [w1266 w1267]
              tunnel: [w1266 w1267] -> w1264
              tunnel: w1255 -> [_ w1269]
              tunnel: w1263 -> [_ w1268]
              frame False {
              }
              frame True {
                n530 = call "Scripting_ReplaceGoop2OORef.vi"("ViRef"=w1269, "Classes(.lvclass files)"=w1268, "error in (no error)"=w1267) -> ()  [unwired: 16 in, 1 out]
              }
            }
          }
          n531 = Format Into String(format string="Updating GOOP Ref: %s", w1236) -> (resulting string=w1235:string)  [unwired: 2 in, 1 out]
          n532 = property on="Progress" class="LstBox (strict)"() -> ("Item Names"=w1245:string[], "Number of Rows"=w1239:u32)  [unwired: 2 in, 2 out]
          n533 = Build Array (concatenate)(w1245, w1235) -> (w1240:string[])
          n534 = Array Size(array=w1240) -> (size(s)=w1244:i32)
          n535 = Subtract(x=w1244, y=w1239) -> (x-y=w1243:u32)
          n536 = To Long Integer(number=w1243) -> (32bit integer=w1241:i32)
          n537 = Max & Min(x=w1241, y=0) -> (max(x,y)=w1238:i32)  [unwired: 1 out]
          n538 = property on="Progress" class="LstBox (strict)"("Item Names"=w1240, "Top Row"=w1238) -> ()  [unwired: 2 in, 2 out]
          n539 = stacked-sequence {
            tunnel: w1234 -> [_]
            frame #0 {
              n540 = Wait (ms)(milliseconds to wait=u32 5) -> ()  [unwired: 1 out]
            }
          }
        }
        n541 = Unbundle By Name(w1212) -> ("VIsToRelink"=w1216:refnum<vi>[])
        n542 = for {
          shift-right: [w1221] -> w1214
          shift-left: w1217 -> [w1225]
          tunnel: w1216 -> [w1224] mode=indexing
          tunnel: w1215 -> [w1222]
          n543 = Not A Number/Path/Refnum?(number/path/refnum=w1224) -> (NaN/Path/Refnum?=w1223:bool)
          n544 = case shown="False" w1223 {
            tunnel: w1225 -> [w1229 w1230]
            tunnel: [w1229 w1230] -> w1221
            tunnel: w1224 -> [w1228 _]
            tunnel: w1222 -> [w1227 _]
            frame False {
              n545 = call "Scripting_ReplaceGoop2OORef.vi"("ViRef"=w1228, "Classes(.lvclass files)"=w1227, "error in (no error)"=w1229) -> ()  [unwired: 16 in, 1 out]
            }
            frame True {
            }
          }
          n546 = stacked-sequence {
            tunnel: w1221 -> [_]
            frame #0 {
              n547 = Wait (ms)(milliseconds to wait=u32 5) -> ()  [unwired: 1 out]
            }
          }
        }
        n548 = call "ConvertGoop2ToGoop3_RecompileAll.vi"("error IO 2"=w1214, "Cluster 2"=w1212) -> ("error IO"=w1213:errorcluster)  [unwired: 7 in]
      }
      frame "UpdateCreate" {
        n549 = Unbundle By Name(w1271) -> ("Classes"=w1276:T2[])
        n550 = for {
          tunnel: w1276 -> [w1302] mode=indexing
          shift-right: [w1290] -> w1275
          shift-left: w1277 -> [w1304]
          tunnel: [w1306] -> w1273 mode=indexing
          n551 = Unbundle By Name(w1302) -> ("ViRefs"=w1305:refnum<vi>[], "ClassName"=w1291:string)
          n552 = for {
            tunnel: w1305 -> [w1315] mode=indexing
            shift-right: [w1316] -> w1303
            shift-left: w1304 -> [w1317]
            n553 = call "Scripting_SaveVi.vi"("error in (no error)"=w1317, "VIRefToSaveIn"=w1315) -> ("error out"=w1316:errorcluster)  [unwired: 8 in, 1 out]
          }
          n554 = Unbundle By Name(w1302) -> ("ViRefs"=w1309:refnum<vi>[], "ViPathes"=w1313:path[])  [unwired: 2 out]
          n555 = Format Into String(format string="Updating Create: %s", w1291) -> (resulting string=w1292:string)  [unwired: 2 in, 1 out]
          n556 = for {
            tunnel: w1313 -> [w1326] mode=indexing
            tunnel: "_Create.vi$" ("regular expression") -> [w1324]
            tunnel: [w1322] -> w1311 mode=indexing
            n557 = Strip Path(path=w1326) -> (name=w1325:string)  [unwired: 1 out]
            n558 = Match Pattern(string=w1325, regular expression=w1324) -> (offset past match=w1323:i32)  [unwired: 1 in, 3 out]
            n559 = Greater Or Equal To 0?(x=w1323) -> (x >= 0?=w1322:bool)
          }
          n560 = property on="Progress" class="LstBox (strict)"() -> ("Item Names"=w1301:string[], "Number of Rows"=w1295:u32)  [unwired: 2 in, 2 out]
          n561 = Build Array (concatenate)(w1301, w1292) -> (w1296:string[])
          n562 = Array Size(array=w1296) -> (size(s)=w1300:i32)
          n563 = Subtract(x=w1300, y=w1295) -> (x-y=w1299:u32)
          n564 = To Long Integer(number=w1299) -> (32bit integer=w1297:i32)
          n565 = Search 1D Array(1D array=w1311, element=TRUE) -> (index of element=w1308:i32)  [unwired: 1 in]
          n566 = Index Array(array=w1309, index=w1308) -> (element=w1307:refnum<vi>)
          n567 = Max & Min(x=w1297, y=0) -> (max(x,y)=w1294:i32)  [unwired: 1 out]
          n568 = property on="Progress" class="LstBox (strict)"("Item Names"=w1296, "Top Row"=w1294) -> ()  [unwired: 2 in, 2 out]
          n569 = case shown="0, Default" w1308 {
            tunnel: w1303 -> [w1318 w1321]
            tunnel: [w1318 w1321] -> w1290
            tunnel: w1307 -> [w1320 _]
            tunnel: [w1320 _] -> w1306
            frame 0, Default {
              n570 = call "Scripting_UpdateGoop2Create.vi"("ViRef"=w1320, "RemovePreloadDynamicMethods"=FALSE, "error in (no error)"=w1318) -> ()  [unwired: 16 in, 1 out]
            }
            frame -1 {
            }
          }
          n571 = stacked-sequence {
            tunnel: w1290 -> [_]
            frame #0 {
              n572 = Wait (ms)(milliseconds to wait=u32 5) -> ()  [unwired: 1 out]
            }
          }
        }
        n573 = Unbundle By Name(w1271) -> ("AppRef"=w1270:refnum<vi>)
        n574 = for {
          shift-right: [w1281] -> w1274
          shift-left: w1275 -> [w1282]
          tunnel: w1273 -> [w1280] mode=indexing
          tunnel: w1270 -> [w1278]
          n575 = Not A Number/Path/Refnum?(number/path/refnum=w1280) -> (NaN/Path/Refnum?=w1279:bool)
          n576 = case shown="False" w1279 {
            tunnel: path "PreloadDynamicMethods.vi" ("Path") -> [w1288 _]
            tunnel: w1282 -> [w1285 w1289]
            tunnel: [w1285 w1289] -> w1281
            tunnel: w1280 -> [w1287 _]
            tunnel: w1278 -> [w1284 _]
            frame False {
              n577 = call "Scripting_RemoveSubViAndFixWires.vi"("MainViPath/ViRef/BlockDiagramRef"=w1287, "SubVIToRemove"=w1288, "SaveVIBeforeRemove(False)"=TRUE, "error in (no error)"=w1285, "AppRef"=w1284) -> ()  [unwired: 14 in, 1 out]
            }
            frame True {
            }
          }
        }
      }
      frame "UpdateDynamicDispatchVIs" {
        n578 = call "ConvertGoop2ToGoop3_RecompileAll.vi"("error IO 2"=w1329, "Cluster 2"=w1327) -> ("error IO"=w1328:errorcluster)  [unwired: 7 in]
        n579 = Unbundle By Name(w1327) -> ("Classes"=w1334:T2[])
        n580 = for {
          tunnel: w1334 -> [w1338] mode=indexing
          shift-right: [w1336] -> w1335
          shift-left: w1328 -> [w1358]
          tunnel: w1334 -> [w1355]
          shift-right: [w1349] -> w1331
          shift-left: refnum<vi>[] [] -> [w1350]
          i -> [w1354]
          n581 = Unbundle By Name(w1338) -> ("ClassName"=w1337:string)
          n582 = Delete From Array(array=w1355, index=w1354) -> (array with subset deleted=w1353:T2[])  [unwired: 1 in, 1 out]
          n583 = for {
            tunnel: w1353 -> [w1364] mode=indexing
            shift-right: [w1362] -> w1351
            shift-left: string[] [] -> [w1363]
            n584 = Unbundle By Name(w1364) -> ("ViPathes"=w1360:path[])
            n585 = for {
              tunnel: [w1366] -> w1361 mode=indexing
              tunnel: w1360 -> [w1365] mode=indexing
              n586 = Strip Path(path=w1365) -> (name=w1366:string)  [unwired: 1 out]
            }
            n587 = Build Array (concatenate)(w1363, w1361) -> (w1362:string[])
          }
          n588 = Unbundle By Name(w1338) -> ("ViRefs"=w1357:refnum<vi>[], "ViPathes"=w1356:path[])  [unwired: 2 out]
          n589 = Format Into String(format string="Updating dynamic dispatch: %s", w1337) -> (resulting string=w1340:string)  [unwired: 2 in, 1 out]
          n590 = property on="Progress" class="LstBox (strict)"() -> ("Item Names"=w1348:string[], "Number of Rows"=w1342:u32)  [unwired: 2 in, 2 out]
          n591 = Build Array (concatenate)(w1348, w1340) -> (w1343:string[])
          n592 = for {
            shift-right: [w1383] -> w1336
            shift-left: w1358 -> [w1384]
            tunnel: w1357 -> [w1369] mode=indexing
            tunnel: w1356 -> [w1382] mode=indexing
            tunnel: w1351 -> [w1376]
            shift-right: [w1372] -> w1349
            shift-left: w1350 -> [w1371]
            n593 = Strip Path(path=w1382) -> (stripped path=w1381:path, name=w1378:string)
            n594 = To Lower Case(string=w1376) -> (all lower case string=w1375:string[])
            n595 = To Lower Case(string=w1378) -> (all lower case string=w1377:string)
            n596 = Strip Path(path=w1381) -> (name=w1370:string)  [unwired: 1 out]
            n597 = Search 1D Array(1D array=w1375, element=w1377) -> (index of element=w1374:i32)  [unwired: 1 in]
            n598 = Not Equal?(x=w1370, y="utils") -> (x != y?=w1379:bool)
            n599 = Not A Number/Path/Refnum?(number/path/refnum=w1369) -> (NaN/Path/Refnum?=w1367:bool)
            n600 = Greater Or Equal To 0?(x=w1374) -> (x >= 0?=w1373:bool)
            n601 = Compound Arithmetic op=AND(invert w1367, w1379) -> (w1368:bool)
            n602 = case shown="True" w1368 {
              tunnel: w1384 -> [w1386 w1391]
              tunnel: [w1386 w1391] -> w1383
              tunnel: w1369 -> [_ w1388]
              tunnel: w1373 -> [_ w1392]
              tunnel: [w1385 w1390] -> w1372
              tunnel: w1371 -> [w1385 w1389]
              frame False {
              }
              frame True {
                n603 = call "Scripting_RemoveDynamicDispatchInGoop2VIs.vi"("ViRef"=w1388, "ForceDynamicDispatch"=w1392, "error in (no error)"=w1391) -> ("DynamicDispatch"=w1387:bool)  [unwired: 15 in, 1 out]
                n604 = case shown="True" w1387 {
                  tunnel: [w1393 w1396] -> w1390
                  tunnel: w1389 -> [w1393 w1395]
                  tunnel: w1388 -> [_ w1394]
                  frame False {
                  }
                  frame True {
                    n605 = Build Array (concatenate)(w1395, w1394) -> (w1396:refnum<vi>[])
                  }
                }
              }
            }
          }
          n606 = Array Size(array=w1343) -> (size(s)=w1347:i32)
          n607 = Subtract(x=w1347, y=w1342) -> (x-y=w1346:u32)
          n608 = To Long Integer(number=w1346) -> (32bit integer=w1344:i32)
          n609 = Max & Min(x=w1344, y=0) -> (max(x,y)=w1341:i32)  [unwired: 1 out]
          n610 = property on="Progress" class="LstBox (strict)"("Item Names"=w1343, "Top Row"=w1341) -> ()  [unwired: 2 in, 2 out]
          n611 = stacked-sequence {
            tunnel: w1336 -> [_]
            frame #0 {
              n612 = Wait (ms)(milliseconds to wait=u32 5) -> ()  [unwired: 1 out]
            }
          }
        }
        n613 = Bundle By Name(cluster=w1327, "SetToDynamicDispatch"=w1331) -> (w1332:T7)
      }
      frame "ExtraSave" {
        n614 = call "ConvertGoop2ToGoop3_RecompileAll.vi"("error IO 2"=w1409, "Cluster 2"=w1407) -> ("error IO"=w1408:errorcluster)  [unwired: 7 in]
        n615 = property on="Progress" class="LstBox (strict)"() -> ("Item Names"=w1406:string[], "Number of Rows"=w1400:u32)  [unwired: 2 in, 2 out]
        n616 = Build Array (concatenate)(w1406, "Recompiling VIs again") -> (w1401:string[])
        n617 = Array Size(array=w1401) -> (size(s)=w1405:i32)
        n618 = Subtract(x=w1405, y=w1400) -> (x-y=w1404:u32)
        n619 = To Long Integer(number=w1404) -> (32bit integer=w1402:i32)
        n620 = Max & Min(x=w1402, y=0) -> (max(x,y)=w1399:i32)  [unwired: 1 out]
        n621 = property on="Progress" class="LstBox (strict)"("Item Names"=w1401, "Top Row"=w1399) -> ()  [unwired: 2 in, 2 out]
      }
      frame "SetDynamicDispatch" {
        n622 = Unbundle By Name(w1422) -> ("SetToDynamicDispatch"=w1410:refnum<vi>[])
        n623 = property on="Progress" class="LstBox (strict)"() -> ("Item Names"=w1420:string[], "Number of Rows"=w1414:u32)  [unwired: 2 in, 2 out]
        n624 = Build Array (concatenate)(w1420, "Setting dynamic dispatch" ("format string")) -> (w1415:string[])
        n625 = Array Size(array=w1415) -> (size(s)=w1419:i32)
        n626 = Subtract(x=w1419, y=w1414) -> (x-y=w1418:u32)
        n627 = To Long Integer(number=w1418) -> (32bit integer=w1416:i32)
        n628 = Max & Min(x=w1416, y=0) -> (max(x,y)=w1413:i32)  [unwired: 1 out]
        n629 = property on="Progress" class="LstBox (strict)"("Item Names"=w1415, "Top Row"=w1413) -> (error out=w1411:errorcluster)  [unwired: 2 in, 1 out]
        n630 = for {
          N -> [w1425]
          tunnel: w1410 -> [w1428] mode=indexing
          tunnel: w1411 -> [_]
          i -> [w1426]
          n631 = Not A Number/Path/Refnum?(number/path/refnum=w1428) -> (NaN/Path/Refnum?=w1427:bool)
          n632 = Increment(x=w1426) -> (x+1=w1424:i32)
          n633 = case shown="False" w1427 {
            tunnel: w1428 -> [w1433 _]
            tunnel: w1424 -> [w1430 _]
            tunnel: w1425 -> [w1429 _]
            frame False {
              n634 = property class="VI"(reference=w1433) -> (error out=w1441:errorcluster, "ConPane"=w1439:refnum<vi>, "Path"=w1438:path)  [unwired: 1 in, 1 out]
              n635 = Strip Path(path=w1438) -> (stripped path=w1437:path, name=w1432:string)
              n636 = stacked-sequence {
                tunnel: w1432 -> [w1442]
                tunnel: [w1442] -> w1431
                frame #0 {
                  w1446 = path "c:/G2To3.txt" ("file (use dialog)")
                  n637 = Read from Text File(file (use dialog)=w1446) -> (text=w1443:string)  [unwired: 3 in, 3 out]
                  n638 = Concatenate Strings(w1443, w1442, "\n" ("string")) -> (w1444:string)
                  n639 = stacked-sequence {
                    tunnel: w1444 -> [w1449]
                    tunnel: w1446 -> [w1447]
                    frame #0 {
                      n640 = Delete(path (use dialog)=w1447) -> (deleted path=w1448:path)  [unwired: 4 in, 2 out]
                      n641 = Write to Text File(file (use dialog)=w1448, text=w1449) -> ()  [unwired: 2 in, 3 out]
                    }
                  }
                }
              }
              n642 = Strip Path(path=w1437) -> (name=w1435:string)  [unwired: 1 out]
              n643 = Not Equal?(x=w1435, y="private") -> (x != y?=w1434:bool)
              n644 = case shown="True" w1434 {
                tunnel: w1441 -> [_ w1469]
                tunnel: [w1450 w1468] -> w1440
                tunnel: w1439 -> [w1450 w1466]
                tunnel: w1431 -> [_ w1455]
                tunnel: w1430 -> [_ w1453]
                tunnel: w1429 -> [_ w1452]
                frame False {
                }
                frame True {
                  w1467 = T14."Dynamic Dispatch" ("Rule")
                  n645 = Not Equal?(x="Destroy.vi", y=w1455) -> ()  [unwired: 1 out]
                  n646 = Format Into String(format string="Setting dynamic dispatch: %d of %d (%s)", w1453, w1452, w1455) -> (resulting string=w1460:string)  [unwired: 2 in, 1 out]
                  n647 = invoke class="ConPane" method="SetWireRule"(reference=w1466, error in=w1469, "TermIdx"=u32 0 ("Terminal Index"), "Rule"=w1467) -> (reference out=w1463:refnum<vi>, error out=w1464:errorcluster)  [unwired: 1 in, 3 out]
                  n648 = property on="Progress" class="LstBox (strict)" props=["Item Names", "Number of Rows"]() -> ("Item Names"=w1459:string[])  [unwired: 2 in, 3 out]
                  n649 = Array Size(array=w1459) -> (size(s)=w1458:i32)
                  n650 = Decrement(x=w1458) -> (x-1=w1457:i32)
                  n651 = Replace Array Subset(array=w1459, new element=w1460, index=w1457) -> (w1462:string[])
                  n652 = case shown="True" TRUE {
                    tunnel: [w1471 w1477] -> w1468
                    tunnel: w1467 -> [_ w1476]
                    tunnel: w1464 -> [w1470 w1474]
                    tunnel: w1463 -> [w1471 w1473]
                    tunnel: [w1470 w1472] -> w1456
                    frame False {
                    }
                    frame True {
                      n653 = invoke class="ConPane" method="SetWireRule"(reference=w1473, error in=w1474, "TermIdx"=u32 14 ("Terminal Index"), "Rule"=w1476) -> (reference out=w1477:refnum<vi>, error out=w1472:errorcluster)  [unwired: 1 in, 3 out]
                    }
                  }
                  n654 = property on="Progress" class="LstBox (strict)"("Item Names"=w1462) -> ()  [unwired: 2 in, 2 out]
                  n655 = stacked-sequence {
                    tunnel: w1456 -> [_]
                    frame #0 {
                      n656 = Wait (ms)(milliseconds to wait=u32 5) -> ()  [unwired: 1 out]
                    }
                  }
                }
              }
              n657 = Close Reference(reference=w1440) -> ()  [unwired: 1 in, 1 out]
            }
            frame True {
            }
          }
        }
      }
      frame "UpdateAllCallParentMethods" {
        n658 = Unbundle By Name(w1479) -> ("CallParentMethod"=w1483:cluster{"VIRef":refnum<vi>, "Position":T6}[])
        n659 = call "ConvertGoop2ToGoop3_RecompileAll.vi"("error IO 2"=w1481, "Cluster 2"=w1479) -> ("error IO"=w1480:errorcluster)  [unwired: 7 in]
        n660 = for {
          tunnel: w1483 -> [w1504] mode=indexing
          shift-right: [w1490] -> w1482
          shift-left: w1480 -> [w1498]
          w1492 = 2354 items=[".NET Container"=2125, ".NET Refnum"=3441, "3D Picture Control"=23776, "Absolute Value"=1054, "Access Rights"=1412, "ActiveX Container"=2072, "Add"=3915, "Add 1"=1050, "Add Array Elements"=1903, "Agitator"=3831, "AllSpoll"=1960, "Always Copy"=2400, "And"=1061, "And Array Elements"=1911, "Append True/False String"=1511, "Application Refnum"=3412, "Array"=21608, "Array 1"=3300, "Array Constant"=2070, "Array Max & Min"=1907, "Array Size"=1809, "Array Subset"=2044, "Array To Cluster"=1168, "Array To Spreadsheet String"=1540, "Array of Strings to Path"=1422, "Atmospheric Tank"=21751, "Atmospheric Tank 1"=3070, "Automation Close"=8001, "Automation Open"=8000, "Automation Refnum"=3410, "Avogadro Constant (1/mol)"=23520, "Base 10 Logarithm Of e"=23512, "Bin"=21755, "Bin 1"=3073, "Bluetooth Close Connection"=9148, "Bluetooth Create Listener"=9151, "Bluetooth Discover"=9152, "Bluetooth Network Connection Refnum"=3468, "Bluetooth Open Connection"=9153, "Bluetooth Read"=9149, "Bluetooth Wait On Listener"=9147, "Bluetooth Write"=9150, "Boolean Array To Number"=1815, "Boolean To (0,1)"=1167, "Build Array"=2041, "Build Cluster Array"=2047, "Build Path"=1419, "Build Waveform"=2066, "Bundle"=2049, "Bundle By Name"=2057, "Byte Array To String"=1609, "Byte Stream File Refnum"=3408, "CAN Channel"=21966, "CAN Channel 1"=3340, "CAN Channel 2"=2124, "CAN Channel 3"=21817, "CAN Interface"=3339, "CAN Interface 1"=21815, "CAN Interface 2"=2123, "CAN Interface 3"=21964, "CAN Task"=3470, "CAN Task 1"=3471, "CAN Task 2"=21963, "CAN Task 3"=21789, "Call By Reference Node"=3901, "Call Chain"=1999, "Call Library Function Node"=2062, "Call Parent Method"=2354, "Cancel Button"=21739, "Cancel Notification"=9107, "Carriage Return Constant"=23500, "Case Structure"=2001, "Cast Unit Bases"=1079, "Check Valve"=3833, "Checkbox"=3117, "Class Specifier Constant"=2094, "Classic Radio Buttons"=22003, "Close File"=8052, "Close File 1"=1405, "Close Reference"=8011, "Cluster"=21607, "Cluster 1"=3400, "Cluster Constant"=2071, "Cluster To Array"=1169, "Code Interface Node"=2050, "Coerce To Type"=2402, "Color Box"=3013, "Color Box Constant"=2120, "Color Box Thin Border"=2905, "Color Ramp"=3022, "Combo Box"=3304, "Combo Box 1"=21604, "Combo Box Constant"=2088, "Complex Conjugate"=1048, "Complex To Polar"=1045, "Complex To Re/Im"=1044, "Compound Arithmetic"=2200, "Compressor"=3832, "Concatenate Strings"=2040, "Conditional Disable Structure"=2064, "Constructor Node"=3904, "Control Help Window"=1353, "Control Online Help"=1355, "Control Refnum"=3419, "Convert Unit"=2059, "Conveyer"=3827, "Copy"=8053, "Copy 1"=1416, "Cosecant"=1204, "Cosine"=1201, "Cotangent"=1205, "Create Folder"=8055, "Create User Event"=2073, "Current VI's Menubar"=9000, "Current VI's Path"=1426, "DAQmx Analog Trigger Source"=21774, "DAQmx Analog Trigger Source 1"=3336, "DAQmx Analog Trigger Source 2"=2119, "DAQmx Analog Trigger Source 3"=21951, "DAQmx Device Name"=3318, "DAQmx Device Name 1"=21773, "DAQmx Device Name 2"=21950, "DAQmx Device Name 3"=2093, "DAQmx Global Channel"=3430, "DAQmx Global Channel 1"=3443, "DAQmx Global Channel 2"=21770, "DAQmx Global Channel 3"=21957, "DAQmx Physical Channel"=21777, "DAQmx Physical Channel 1"=3335, "DAQmx Physical Channel 2"=21954, "DAQmx Physical Channel 3"=2118, "DAQmx Scale Name"=2116, "DAQmx Scale Name 1"=21952, "DAQmx Scale Name 2"=21775, "DAQmx Scale Name 3"=3317, "DAQmx Switch"=21776, "DAQmx Switch 1"=21953, "DAQmx Switch 2"=3337, "DAQmx Switch 3"=2121, "DAQmx Task Name"=21778, "DAQmx Task Name 1"=3442, "DAQmx Task Name 2"=3434, "DAQmx Task Name 3"=21959, "DAQmx Terminal"=3319, "DAQmx Terminal 1"=21955, "DAQmx Terminal 2"=2117, "DAQmx Terminal 3"=21781, "Data Log File Refnum"=3402, "DataSocket Close"=1085, "DataSocket Open"=1084, "DataSocket Read"=1086, "DataSocket Refnum"=3417, "DataSocket Write"=1087, "Date/Time To Seconds"=1308, "Decimal Digit?"=1119, "Decimal String To Number"=1184, "Decimate 1D Array"=2046, "Decrement"=1058, "Default Directory"=1427, "Delete"=1417, "Delete 1"=8056, "Delete From Array"=3912, "Delete Menu Items"=9004, "Delete Variant Attribute"=8206, "Delete Waveform Attribute"=8209, "Deny Access"=8057, "Dequeue Element"=9113, "Destroy User Event"=2075, "DevClear"=1961, "DevClearList"=1962, "Device Control/Status"=1433, "Device Refnum"=3405, "Diagram Disable Structure"=2054, "Dial"=3050, "Dial 1"=21732, "Digital Data"=3210, "Digital Data 1"=21216, "Digital Waveform Graph"=3502, "Digital Waveform Graph 1"=21718, "Digital Waveform Graph 2"=3511, "Divide"=3918, "Divide 1"=1053, "Dlg CheckBox"=21924, "Dlg Horiz Scrollbar"=21905, "Dlg Numeric"=2100, "Dlg Numeric 2"=3006, "Dlg String"=2110, "Dlg Vert Scrollbar"=21906, "Down Arrow"=3824, "Down Bow Valve"=3807, "Down Bow Valve 1"=21767, "Down Bow Valve 2"=3707, "Down Rect Valve"=21766, "Down Rect Valve 1"=3806, "Down Rect Valve 2"=3706, "Down Tee"=3718, "Down Tee 1"=3818, "EOF"=1410, "Elementary Charge (C)"=23517, "Empty Array?"=23063, "Empty Path Constant"=23523, "Empty String Constant"=23503, "Empty String/Path?"=1112, "Empty Variant"=8200, "Enable Menu Tracking"=9002, "EnableLocal"=1963, "EnableRemote"=1964, "End of Line Constant"=23525, "Enqueue Element"=9111, "Enqueue Element At Opposite End"=9129, "Enum"=3023, "Enum 1"=21605, "Enum Constant"=2090, "Equal To 0?"=1113, "Equal?"=1102, "Error Ring Constant"=2039, "Event Callback Refnum"=3435, "Event Data Node"=2102, "Event Structure"=2052, "Exchanger"=3828, "Exclusive Or"=1063, "Exponential"=1211, "Exponential (Arg) -1"=1222, "Expression Node"=2201, "False Constant"=2006, "Feedback Node"=2353, "FieldPoint IO Point"=3440, "FieldPoint IO Point 1"=21784, "FieldPoint IO Point 2"=3439, "File Dialog"=8081, "File Dialog 1"=8058, "File Path Control"=3203, "File Path Control 1"=21730, "File Path Indicator"=3204, "File Path Indicator 1"=21731, "File/Directory Info"=8082, "File/Directory Info 1"=1413, "FindLstn"=1965, "FindRQS"=1966, "First Call?"=1083, "Flat Box"=3602, "Flat Circle"=3605, "Flat Down Triangle"=3623, "Flat Frame"=3608, "Flat Left Triangle"=3620, "Flat Right Triangle"=3621, "Flat Round Button"=3102, "Flat Rounded Box"=3611, "Flat Sequence Structure"=2069, "Flat Square Button"=3103, "Flat Up Triangle"=3622, "Flatten To String"=1164, "Flatten To XML"=8400, "Flattened String To Variant"=8202, "Floating Point Equal?"=23064, "Flush File"=1406, "Flush File 1"=8059, "Flush Queue"=9114, "For Loop"=2002, "Format Date/Time String"=8100, "Format Into File"=2083, "Format Into String"=2081, "Format Value"=1512, "Formula Node"=2004, "Fract/Exp String To Number"=1187, "Framed Color Box"=21019, "Framed Color Box 1"=3008, "Free Label"=2321, "Furnace"=3829, "GPIB Clear"=1954, "GPIB Initialization"=1957, "GPIB Misc"=1956, "GPIB Read"=1951, "GPIB Serial Poll"=1955, "GPIB Status"=1959, "GPIB Trigger"=1953, "GPIB Wait"=1958, "GPIB Write"=1950, "Gauge"=21009, "Gauge 1"=3040, "Generate Front Panel Activity"=1329, "Generate Occurrence"=1700, "Generate User Event"=2074, "Get Datalog Position"=8061, "Get Date/Time In Seconds"=1303, "Get Date/Time String"=1600, "Get Drag Drop Data"=9154, "Get File Position"=8062, "Get File Size"=8063, "Get Help Window Status"=1354, "Get Menu Item Info"=9005, "Get Menu Selection"=9001, "Get Menu Short Cut Info"=9007, "Get Notifier Status"=9103, "Get Number of Records"=8064, "Get Permissions"=8065, "Get Queue Status"=9110, "Get Type and Creator"=8066, "Get Variant Attribute"=8205, "Get Volume Info"=8067, "Get Waveform Attribute"=8208, "Get Waveform Components"=2067, "Global Variable"=2060, "Gravitational Constant (N m2/kg2)"=23519, "Greater Or Equal To 0?"=1114, "Greater Or Equal?"=1103, "Greater Than 0?"=1117, "Greater?"=1110, "Handle Peek"=1604, "Handle Poke"=1605, "Hex Digit?"=1123, "Hexadecimal String To Number"=1185, "Hopper"=3072, "Hopper 1"=21754, "Horiz Line"=3821, "Horiz Pipe"=3710, "Horiz Pipe 1"=3810, "Horizontal Button Box"=3636, "Horizontal Fill Slide"=21100, "Horizontal Fill Slide 1"=3012, "Horizontal Graduated Bar"=21106, "Horizontal Pointer Slide"=3011, "Horizontal Pointer Slide 1"=21101, "Horizontal Progress Bar"=21102, "Horizontal Scrollbar"=21110, "Horizontal Slide"=3010, "Horizontal Slide Switch"=3114, "Horizontal Smooth Box"=3633, "Horizontal Splitter Bar"=21861, "Horizontal Splitter Bar (Classic)"=21863, "Horizontal Splitter Bar (System)"=21865, "Horizontal Switch"=3108, "Horizontal Tank"=3071, "Horizontal Toggle Switch"=21700, "Horizontal Toggle Switch 1"=3110, "Hyperbolic Cosecant"=23053, "Hyperbolic Cosine"=1215, "Hyperbolic Cotangent"=23055, "Hyperbolic Secant"=23054, "Hyperbolic Sine"=1214, "Hyperbolic Tangent"=1216, "IMAQ Session"=3415, "IP To String"=1710, "IVI Delete Session"=8103, "IVI Logical Name"=3414, "IVI Logical Name 1"=21736, "IVI Logical Name 2"=3420, "IVI New Session"=8102, "Implies"=1080, "In Range and Coerce"=1127, "Increment"=1057, "Index & Bundle Cluster Array"=2056, "Index Array"=2042, "Index String Array"=1531, "Initialize Array"=2053, "Inline C Node"=2104, "Input"=1351, "Insert Into Array"=3911, "Insert Menu Items"=9003, "Intensity Chart"=3509, "Intensity Chart 1"=21719, "Intensity Graph"=3510, "Intensity Graph 1"=21720, "Interleave 1D Arrays"=2045, "Interpolate 1D Array"=1905, "Inverse Cosecant"=23050, "Inverse Cosine"=1207, "Inverse Cotangent"=23052, "Inverse Hyperbolic Cosecant"=23056, "Inverse Hyperbolic Cosine"=1218, "Inverse Hyperbolic Cotangent"=23058, "Inverse Hyperbolic Secant"=23057, "Inverse Hyperbolic Sine"=1217, "Inverse Hyperbolic Tangent"=1219, "Inverse Secant"=23051, "Inverse Sine"=1206, "Inverse Tangent"=1208, "Inverse Tangent (2 Input)"=1228, "Invoke Node"=3900, "IrDA Close Connection"=9144, "IrDA Create Listener"=9140, "IrDA Discover"=9141, "IrDA Network Connection Refnum"=3450, "IrDA Open Connection"=9142, "IrDA Read"=9145, "IrDA Wait On Listener"=9143, "IrDA Write"=9146, "Join Numbers"=1171, "Knob"=3005, "Knob 1"=21000, "LED Button"=3116, "LabVIEW Object"=3457, "Label"=21960, "Labeled Oblong Button"=3125, "Labeled Rectangular Button"=3124, "Labeled Round Button"=3122, "Labeled Square Button"=3123, "Left Arrow"=3826, "Left Bow Valve"=3801, "Left Bow Valve 1"=3701, "Left Bow Valve 2"=21761, "Left Down Elbow"=3711, "Left Down Elbow 1"=3811, "Left Pump"=3713, "Left Pump 1"=3813, "Left Rect Valve"=3800, "Left Rect Valve 1"=21760, "Left Rect Valve 2"=3700, "Left Tee"=3709, "Left Tee 1"=3809, "Left Up Elbow"=3808, "Left Up Elbow 1"=3708, "Less Or Equal To 0?"=1115, "Less Or Equal?"=1104, "Less Than 0?"=1118, "Less?"=1111, "Lexical Class"=1126, "Line Feed Constant"=23501, "List Directory"=1418, "List Folder"=8083, "Listbox"=21806, "Listbox 1"=21792, "Listbox Symbol Ring Constant"=2038, "Local Variable"=2061, "Lock Range"=1411, "Logarithm Base 10"=1210, "Logarithm Base 2"=1225, "Logarithm Base X"=1224, "Logical Shift"=1081, "Lookup Table Refnum"=3426, "Lowered Rounded Box"=3638, "MATLAB Script Node"=9020, "Machine Epsilon"=23528, "MakeAddr"=1967, "Mantissa & Exponent"=1150, "Match First String"=1532, "Match Pattern"=1535, "Match True/False String"=1533, "MathScript Node"=2357, "Max & Min"=1108, "Menu Refnum"=3413, "Menu Ring"=3018, "Menu Ring 1"=21600, "Menu-Popup Ring"=3017, "Merge Signals"=2350, "Meter"=21008, "Meter 1"=3030, "Mixed Signal Graph"=21721, "Molar Gas Constant (J/(mol K))"=23522, "Motion Resource"=3449, "Motion Resource 1"=21787, "Motion Resource 2"=3448, "Motor"=3820, "Motor 1"=3720, "Move"=1415, "Move 1"=8068, "Multicolumn Listbox"=21791, "Multicolumn Listbox 1"=21799, "Multiple Selection Listbox"=3208, "Multiply"=3917, "Multiply 1"=1052, "Multiply Array Elements"=1904, "Multirate Structure"=2199, "Natural Logarithm"=1209, "Natural Logarithm (Arg +1)"=1221, "Natural Logarithm Base"=23510, "Natural Logarithm Of 10"=23513, "Natural Logarithm Of 2"=23514, "Natural Logarithm Of Pi"=23508, "Negate"=1069, "Negative Infinity"=23509, "New Directory"=1402, "New File"=1404, "New VI"=8014, "New VI Object"=8015, "Not"=1064, "Not A Number/Path/Refnum?"=1128, "Not A Path Constant"=23524, "Not And"=1071, "Not Equal To 0?"=1116, "Not Equal?"=1105, "Not Exclusive Or"=1073, "Not Or"=1072, "Not a Refnum Constant"=23526, "Not a Shared Variable"=23527, "Notifier Refnum"=3423, "Number To Boolean Array"=1814, "Number To Decimal String"=1180, "Number To Engineering String"=1183, "Number To Exponential String"=1505, "Number To Fractional String"=1506, "Number To Hexadecimal String"=1181, "Number To Octal String"=1182, "Numeric Constant"=2005, "Numeric Control"=3000, "Numeric Control 1"=21003, "Numeric Indicator"=3001, "Numeric Indicator 1"=21004, "OK Button"=21738, "OLE Variant"=3150, "Obtain Notifier"=9101, "Obtain Queue"=9108, "Occurrence Refnum"=3406, "Octal Digit?"=1129, "Octal String To Number"=1186, "Old VISA Open"=1921, "One Button Dialog"=1340, "Open Application Reference"=8012, "Open Device"=1430, "Open File"=1403, "Open Tank"=21752, "Open Tank 1"=3074, "Open VI Object Reference"=8013, "Open VI Reference"=8010, "Open/Create/Replace Datalog"=8054, "Open/Create/Replace File"=8050, "Or"=1062, "Or Array Elements"=1910, "PPoll"=1969, "PPollConfig"=1970, "PPollUnconfig"=1971, "Package Matrix"=23001, "PassControl"=1968, "Path Constant"=2009, "Path To String"=1077, "Path Type"=1421, "Path to Array of Strings"=1423, "Pi"=23504, "Pi Divided By 2"=23506, "Pi Multiplied By 2"=23505, "Pick Line"=1510, "Pict Ring"=3015, "Pict Ring 1"=21602, "Picture"=3508, "PixMap"=3505, "PixMap (Do not touch it!!)"=3507, "Planck Constant (J/Hz)"=23516, "Platform Flat Square Button"=3134, "Plug-In Control"=21820, "Polar To Complex"=1047, "Polar To Re/Im"=23061, "Positive Infinity"=23515, "Power Of 10"=1212, "Power Of 2"=1223, "Power Of X"=1213, "Pressure Tank"=21753, "Pressure Tank 1"=3075, "Preview Queue Element"=9112, "Printable?"=1124, "Priority Queue Refnum"=3425, "Property Node"=1920, "Pulldown Menu Ring"=3061, "Push Button"=21001, "Queue Refnum"=3474, "Queue Refnum 1"=3424, "Quit LabVIEW"=1352, "Quotient & Remainder"=1056, "RT FIFO Create"=24000, "RT FIFO Delete"=24003, "RT FIFO Read"=24001, "RT FIFO Write"=24002, "Radio Buttons"=22001, "Raised Box"=3637, "Raised Box 1"=3600, "Raised Circle"=3603, "Raised Down Triangle"=3615, "Raised Frame"=3606, "Raised Left Triangle"=3612, "Raised Right Triangle"=3613, "Raised Rounded Box"=3609, "Raised Up Triangle"=3614, "Random Number (0-1)"=1070, "RcvRespMsg"=1972, "Re/Im To Complex"=1046, "Re/Im To Polar"=23060, "Read Datalog"=8069, "Read Device"=1432, "Read File"=1407, "Read from Binary File"=8051, "Read from Text File"=8070, "ReadStatus"=1973, "Receive"=1974, "ReceiveSetup"=1975, "Recessed Box"=3601, "Recessed Circle"=3604, "Recessed Down Triangle"=3619, "Recessed Frame"=3607, "Recessed Left Triangle"=3616, "Recessed Menu Ring"=3019, "Recessed Right Triangle"=3617, "Recessed Rounded Box"=3610, "Recessed Up Triangle"=3618, "Reciprocal"=1059, "Reciprocal Of Pi"=23507, "Reciprocal Of e"=23511, "Rectangular Stop Button"=3128, "Refnum to Path"=1424, "Refnum to Session"=2306, "Register Event Callback"=2078, "Register For Events"=2065, "Register Session"=2319, "Release Notifier"=9102, "Release Queue"=9109, "Replace Array Subset"=3910, "Replace Substring"=3913, "Request Deallocation"=1610, "ResetSys"=1976, "Reshape Array"=2055, "Reverse 1D Array"=1900, "Reverse String"=1537, "Right Arrow"=3825, "Right Bow Valve"=21765, "Right Bow Valve 1"=3805, "Right Bow Valve 2"=3705, "Right Down Elbow"=3717, "Right Down Elbow 1"=3817, "Right Pump"=3819, "Right Pump 1"=3719, "Right Rect Valve"=3704, "Right Rect Valve 1"=3804, "Right Rect Valve 2"=21764, "Right Tee"=3815, "Right Tee 1"=3715, "Right Up Elbow"=3714, "Right Up Elbow 1"=3814, "Ring Constant"=2008, "Rocker"=21002, "Rotary Feeder"=3830, "Rotate"=1082, "Rotate 1D Array"=1906, "Rotate Left With Carry"=1606, "Rotate Right With Carry"=1607, "Rotate String"=1536, "Round Button"=3100, "Round LED"=3120, "Round LED 1"=21012, "Round Light"=3104, "Round Push Button"=3112, "Round Push Button 2"=3118, "Round Radio Button"=3106, "Round Stop Button"=3127, "Round To +Infinity"=1076, "Round To -Infinity"=1075, "Round To Nearest"=1055, "Rydberg Constant (1/m)"=23521, "Scale By Power Of 2"=1074, "Scan From File"=2082, "Scan From String"=2080, "Scan String For Tokens"=8101, "Scan Value"=1534, "Search 1D Array"=1901, "Search and Replace String"=3914, "Search/Split String"=1538, "Secant"=1203, "Seconds To Date/Time"=1309, "Seek"=1409, "Select"=1516, "Send"=1977, "Send Notification"=9104, "SendCmds"=1978, "SendDataBytes"=1979, "SendIFC"=1980, "SendLLO"=1982, "SendList"=1981, "SendSetup"=1983, "Session to Refnum"=2307, "Set Datalog Position"=8072, "Set File Position"=8073, "Set File Size"=8074, "Set Menu Item Info"=9006, "Set Number of Records"=8075, "Set Occurrence"=1702, "Set Permissions"=8076, "Set Type and Creator"=8077, "Set Variant Attribute"=8204, "Set Waveform Attribute"=8207, "SetRWLS"=1984, "SetTimeOut"=1985, "Shared Variable Constant"=3473, "Shared Variable Control"=21814, "Shared Variable Control 1"=3472, "Shared Variable to String"=1831, "Sign"=1049, "Simple Horizontal Slide"=3003, "Simple Numeric"=3029, "Simple Numeric 1"=2900, "Simple String"=2115, "Simple Vertical Slide"=3002, "Simulation Loop"=2099, "Sinc"=1227, "Sine"=1200, "Sine & Cosine"=1220, "Size Handle"=1603, "Slide Switch"=21011, "Sort 1D Array"=1120, "Sort Array of String, Sort Array of String 1"=23065, "Speed Of Light In Vacuum (m/sec)"=23518, "Split 1D Array"=1908, "Split Button"=21020, "Split Number"=1170, "Split Signals"=2351, "Spreadsheet String To Array"=1539, "Square"=23059, "Square Button"=3101, "Square LED"=3121, "Square LED 1"=21013, "Square Light"=3105, "Square Push Button"=3113, "Square Push Button 2"=3119, "Square Radio Button"=3107, "Square Root"=1060, "Stacked Sequence Structure"=2000, "State Diagram"=2051, "Static VI Reference"=2084, "Stop"=1350, "Stop Button"=21230, "String Constant"=2007, "String Control"=21701, "String Control 1"=3200, "String Indicator"=21702, "String Indicator 1"=3201, "String Length"=1502, "String Subset"=1503, "String To Byte Array"=1608, "String To IP"=1711, "String To Path"=1078, "String to Shared Variable"=1830, "Strip Path"=1420, "SubPanel"=21810, "SubPanel (Classic)"=21811, "Subtract"=3916, "Subtract 1"=1051, "Swap Bytes"=1162, "Swap Values"=2401, "Swap Vector Element"=1912, "Swap Words"=1163, "System Button"=3130, "System Cancel Button"=3131, "System Checkbox"=3132, "System Chiseled Line"=3632, "System Colored Rectangle"=3625, "System Combo Box"=21917, "System Enum"=3062, "System Horizontal Pointer Slide"=21902, "System Horizontal Progress Bar"=21910, "System Horizontal Slide"=21904, "System Label"=21961, "System Listbox"=21805, "System Multicolumn Listbox"=21798, "System Numeric"=21919, "System Path Control"=21922, "System Pict Ring"=21925, "System Radio Button"=3133, "System Radio Buttons"=22002, "System Recessed Frame"=3624, "System Ring"=3060, "System Spin Control"=21900, "System String"=21920, "System Tab Control"=3331, "System Table"=21797, "System Time Stamp"=21967, "System Tree"=21794, "System Vertical Pointer Slide"=21901, "System Vertical Progress Bar"=21909, "System Vertical Slide"=21903, "TCP Close Connection"=1713, "TCP Create Listener"=1717, "TCP Flattened Read"=1718, "TCP Flattened Write"=1719, "TCP Flex Read"=1720, "TCP Flex Write"=1721, "TCP Network Connection Refnum"=3407, "TCP Open Connection"=1715, "TCP Read"=1716, "TCP Wait On Listener"=1712, "TCP Write"=1714, "TDMS Close"=2013, "TDMS Defragment"=2019, "TDMS File"=3477, "TDMS Flush"=2017, "TDMS Get Properties"=2015, "TDMS List Contents"=2016, "TDMS Open"=2012, "TDMS Read"=2011, "TDMS Set Properties"=2014, "TDMS Write"=2010, "TDMS Write IP"=2018, "Tab Constant"=23502, "Tab Control"=3332, "Tab Control 1"=3330, "Table"=21796, "Table 1"=21790, "Tag Attribute Ring"=2063, "Tag Constant"=2089, "Tag Control"=3302, "Tag Control 1"=21742, "Tag Indicator"=3303, "Tag Indicator 1"=21743, "Tangent"=1202, "Tank"=21006, "Tank 1"=3020, "Temporary Directory"=1435, "TestSRQ"=1986, "TestSys"=1987, "Text & Pict Ring"=21603, "Text & Pict Ring 1"=3016, "Text Button"=21015, "Text Ring"=21601, "Text Ring 1"=3014, "Text to UTF-8"=23066, "Thermometer"=21007, "Thermometer 1"=3021, "Thick Chiseled Line"=3630, "Thick Line"=3629, "Thick Line with Arrow"=3631, "Thick Lowered Box"=3635, "Thin Chiseled Line"=3627, "Thin Line"=3626, "Thin Line with Arrow"=3628, "Threshold 1D Array"=1909, "Tick Count (ms)"=1300, "Time Stamp Constant"=2068, "Time Stamp Control"=5555, "Time Stamp Control 1"=21913, "Time Stamp Indicator"=5556, "Time Stamp Indicator 1"=21914, "Timed Loop"=5570, "Timed Sequence"=5573, "To Byte Integer"=1140, "To Double Precision Complex"=1152, "To Double Precision Float"=1147, "To Extended Precision Complex"=1154, "To Extended Precision Float"=1149, "To Long Integer"=1142, "To Lower Case"=1189, "To More Generic Class"=8017, "To More Specific Class"=8016, "To OLE Variant"=8002, "To Quad Integer"=1155, "To Single Precision Complex"=1151, "To Single Precision Float"=1146, "To Time Stamp"=5560, "To Unsigned Byte Integer"=1143, "To Unsigned Long Integer"=1145, "To Unsigned Quad Integer"=1156, "To Unsigned Word Integer"=1144, "To Upper Case"=1188, "To Variant"=8201, "To Word Integer"=1141, "Traditional DAQ Channel"=21733, "Traditional DAQ Channel 1"=3320, "Traditional DAQ Channel 2"=2085, "Transpose 2D Array"=1902, "Tree"=21819, "Tree 1"=21793, "Trigger"=1988, "TriggerList"=1989, "Two Button Dialog"=1341, "Type Cast"=1166, "Type and Creator"=1434, "UDP Close"=1726, "UDP Multicast Open"=1727, "UDP Network Connection Refnum"=3418, "UDP Open"=1723, "UDP Read"=1724, "UDP Write"=1725, "UTF-8 to Text"=23067, "Unbundle"=2048, "Unbundle By Name"=2058, "Unflatten From String"=1165, "Unflatten From XML"=8401, "Unpackage Matrix"=23000, "Unregister For Events"=2076, "Unregister Session"=2320, "Up Arrow"=3823, "Up Bow Valve"=21763, "Up Bow Valve 1"=3803, "Up Bow Valve 2"=3703, "Up Rect Valve"=3702, "Up Rect Valve 1"=3802, "Up Rect Valve 2"=21762, "Up Tee"=3712, "Up Tee 1"=3812, "User Defined Refnum"=3428, "User Defined Refnum Tag"=3429, "User Defined Refnum Tag 1"=21745, "User Defined Refnum Tag Flatten"=3454, "User Defined Refnum Tag Flatten 1"=21747, "User Defined Tag"=2114, "User Defined Tag 1"=21749, "User Item"=3506, "VI Library"=1425, "VI Refnum"=3422, "VI Server Reference"=2091, "VISA Assert Interrupt Signal"=2309, "VISA Assert Trigger"=1929, "VISA Assert Utility Signal"=2310, "VISA Clear"=1927, "VISA Close"=1922, "VISA Disable Event"=1940, "VISA Discard Events"=1941, "VISA Enable Event"=1942, "VISA Find Resource"=1923, "VISA Flush I/O Buffer"=2302, "VISA GPIB Command"=2315, "VISA GPIB Control ATN"=2316, "VISA GPIB Control REN"=2304, "VISA GPIB Pass Control"=2317, "VISA GPIB Send IFC"=2318, "VISA In 16"=1930, "VISA In 32"=1944, "VISA In 8"=1936, "VISA Lock"=1993, "VISA Map Address"=1932, "VISA Map Trigger"=2311, "VISA Memory Allocation"=1997, "VISA Memory Free"=1998, "VISA Move"=2303, "VISA Move In 16"=1948, "VISA Move In 32"=1991, "VISA Move In 8"=1946, "VISA Move Out 16"=1949, "VISA Move Out 32"=1992, "VISA Move Out 8"=1947, "VISA Open"=2308, "VISA Out 16"=1931, "VISA Out 32"=1945, "VISA Out 8"=1937, "VISA Peek 16"=1934, "VISA Peek 32"=1995, "VISA Peek 8"=1938, "VISA Poke 16"=1935, "VISA Poke 32"=1996, "VISA Poke 8"=1939, "VISA Read"=1925, "VISA Read STB"=1928, "VISA Read To File"=2313, "VISA Refnum to Session"=2300, "VISA Resource Name"=21737, "VISA Resource Name 1"=3421, "VISA Set I/O Buffer Size"=2301, "VISA Status Description"=1924, "VISA USB Control In"=2086, "VISA USB Control Out"=2087, "VISA Unlock"=1994, "VISA Unmap Address"=1933, "VISA Unmap Trigger"=2312, "VISA VXI Cmd or Query"=2305, "VISA Wait on Event"=1943, "VISA Write"=1926, "VISA Write From File"=2314, "VISA resource name"=3409, "Variant"=3310, "Variant To Data"=8003, "Variant To Flattened String"=8203, "Vert Line"=3822, "Vert Pipe"=3716, "Vert Pipe 1"=3816, "Vert Rocker"=21740, "Vertical Fill Slide"=21014, "Vertical Fill Slide 1"=3009, "Vertical Graduated Bar"=21107, "Vertical Pointer Slide"=21017, "Vertical Pointer Slide 1"=3007, "Vertical Progress Bar"=21104, "Vertical Scrollbar"=21111, "Vertical Slide"=3004, "Vertical Slide Switch"=21741, "Vertical Slide Switch 1"=3115, "Vertical Smooth Box"=3634, "Vertical Splitter Bar"=21860, "Vertical Splitter Bar (Classic)"=21862, "Vertical Splitter Bar (System)"=21864, "Vertical Switch"=3109, "Vertical Toggle Switch"=21005, "Vertical Toggle Switch 1"=3111, "Volume Info"=1414, "Wait (ms)"=1302, "Wait For Activity"=1722, "Wait For Front Panel Activity"=1328, "Wait Until Next ms Multiple"=1327, "Wait for GPIB RQS"=1952, "Wait on Notification"=9105, "Wait on Notification from Multiple"=9106, "Wait on Occurrence"=1701, "WaitSRQ"=1990, "Waveform Chart"=3501, "Waveform Chart 1"=21717, "Waveform Chart 2"=21010, "Waveform Graph"=21703, "Waveform Graph 1"=3504, "While Loop"=2003, "While Loop 1"=2352, "White Space?"=1125, "Write Datalog"=8079, "Write Device"=1431, "Write File"=1408, "Write to Binary File"=8078, "Write to Text File"=8080, "XY Graph"=3500, "XY Graph 1"=21716, "Xmath Script Node"=9022, "Y-th root of X"=23062] ("ExchangeType")
          w1496 = refnum<vi> refnum  # Node
          n661 = Unbundle By Name(w1504) -> ("VIRef"=w1489:refnum<vi>, "Position"=w1485:T6)
          n662 = property class="VI"(reference=w1489) -> ("Path"=w1488:path)  [unwired: 1 in, 2 out]
          n663 = Build Array (concatenate)(path[] [path "Unknown", path ""] ("VIsToSerachFor"), w1488) -> (w1486:path[])
          n664 = call "Scripting_FindVisOnDiagram.vi"("ViRef"=w1489, "VIsToSerachFor/ViName"=w1486, "error in (no error)"=w1498) -> ("VisFound"=w1503:refnum<vi>[], "error out"=w1499:errorcluster)  [unwired: 15 in]
          n665 = for {
            tunnel: w1503 -> [w1509] mode=indexing
            tunnel: [w1508] -> w1502 mode=indexing
            tunnel: [w1507] -> w1501 mode=indexing
            shift-right: [w1506] -> w1493
            shift-left: w1499 -> [w1505]
            n666 = property class="GObj"(reference=w1509, error in=w1505) -> (reference out=w1507:refnum<vi>, error out=w1506:errorcluster, "Position"=w1508:T6)
          }
          n667 = Search 1D Array(1D array=w1502, element=w1485) -> (index of element=w1500:i32)  [unwired: 1 in]
          n668 = Index Array(array=w1501, index=w1500) -> (element=w1497:refnum<vi>)
          n669 = To More Specific Class(target class=w1496, reference=w1497, error in=w1493) -> (specific class reference=w1495:refnum<vi>, error out=w1494:errorcluster)
          n670 = call "Scripting_ExchangeNodeAndRewire.vi"("Node"=w1495, "ExchangeType"=w1492, "error in (no error)"=w1494) -> ("error out"=w1491:errorcluster)  [unwired: 16 in]
          n671 = call <vilib>:"Clear Errors.vi"("error in (no error)"=w1491) -> ("error out"=w1490:errorcluster)  [unwired: 5 in, 1 out]
        }
      }
      frame "UpdateDestroy" {
        n672 = Unbundle By Name(w1514) -> ("Classes"=w1513:T2[])
        n673 = for {
          tunnel: w1513 -> [w1518] mode=indexing
          shift-right: [w1516] -> w1511
          shift-left: w1515 -> [w1536]
          n674 = Unbundle By Name(w1518) -> ("ViRefs"=w1531:refnum<vi>[], "ViPathes"=w1535:path[])  [unwired: 2 out]
          n675 = Unbundle By Name(w1518) -> ("ClassName"=w1517:string)
          n676 = for {
            tunnel: w1535 -> [w1546] mode=indexing
            tunnel: "destroy.vi$" ("regular expression") -> [w1544]
            tunnel: [w1542] -> w1533 mode=indexing
            n677 = Strip Path(path=w1546) -> (name=w1545:string)  [unwired: 1 out]
            n678 = To Lower Case(string=w1545) -> (all lower case string=w1541:string)
            n679 = Match Pattern(string=w1541, regular expression=w1544) -> (offset past match=w1543:i32)  [unwired: 1 in, 3 out]
            n680 = Greater Or Equal To 0?(x=w1543) -> (x >= 0?=w1542:bool)
          }
          n681 = Search 1D Array(1D array=w1533, element=TRUE) -> (index of element=w1530:i32)  [unwired: 1 in]
          n682 = Index Array(array=w1531, index=w1530) -> (element=w1529:refnum<vi>)
          n683 = case shown="0, Default" w1530 {
            tunnel: w1536 -> [w1538 w1540]
            tunnel: [w1538 w1540] -> w1516
            tunnel: w1529 -> [w1539 _]
            frame 0, Default {
              n684 = call "Scripting_UpdateGoop2Destroy.vi"("ViRef"=w1539, "error in (no error)"=w1538) -> ()  [unwired: 17 in, 1 out]
            }
            frame -1 {
            }
          }
          n685 = Format Into String(format string="Update destory methods: %s", w1517) -> (resulting string=w1520:string)  [unwired: 2 in, 1 out]
          n686 = property on="Progress" class="LstBox (strict)"() -> ("Item Names"=w1528:string[], "Number of Rows"=w1522:u32)  [unwired: 2 in, 2 out]
          n687 = Build Array (concatenate)(w1528, w1520) -> (w1523:string[])
          n688 = Array Size(array=w1523) -> (size(s)=w1527:i32)
          n689 = Subtract(x=w1527, y=w1522) -> (x-y=w1526:u32)
          n690 = To Long Integer(number=w1526) -> (32bit integer=w1524:i32)
          n691 = stacked-sequence {
            tunnel: w1516 -> [_]
            frame #0 {
              n692 = Wait (ms)(milliseconds to wait=u32 5) -> ()  [unwired: 1 out]
            }
          }
          n693 = Max & Min(x=w1524, y=0) -> (max(x,y)=w1521:i32)  [unwired: 1 out]
          n694 = property on="Progress" class="LstBox (strict)"("Item Names"=w1523, "Top Row"=w1521) -> ()  [unwired: 2 in, 2 out]
        }
        n695 = call "ConvertGoop2ToGoop3_RecompileAll.vi"("error IO 2"=w1511) -> ("error IO"=w1510:errorcluster)  [unwired: 8 in]
      }
      frame "UpdateClassInfo" {
        n696 = Unbundle By Name(w1558) -> ("Classes"=w1560:T2[])
        n697 = for {
          tunnel: w1560 -> [w1567] mode=indexing
          shift-right: [w1563] -> w1547
          shift-left: w1559 -> [w1572]
          n698 = Unbundle By Name(w1567) -> ("ClassRef"=w1565:refnum<vi>, "TemplateVersionUsed"=w1564:string)
          n699 = Unbundle By Name(w1567) -> ("InheritsFrom"=w1571:path)
          n700 = property class="LVClassLibrary"(reference=w1565, error in=w1572) -> (reference out=w1579:refnum<vi>, error out=w1580:errorcluster, "Description"=w1578:string)
          n701 = Empty String/Path?(string/path=w1571) -> (empty?=w1570:bool)
          n702 = Select(t=EndevoTemplateNames."BaseTemplate" ("TemplateNames"), s=w1570, f=EndevoTemplateNames."SubTemplate" ("TemplateNames")) -> (s? t:f=w1566:T10)
          n703 = Format Into String(w1566) -> (resulting string=w1577:string)  [unwired: 3 in, 1 out]
          n704 = Format Into String(EndevoProviderName."EndevoGOOP300" ("ProviderName")) -> (resulting string=w1576:string)  [unwired: 3 in, 1 out]
          n705 = Bundle By Name(cluster=T3 {"ClassProviderName"="", "ClassTemplateUsed"="", "ClassTemplateVersion"="", "ClassDescription"="", "PlugIns"=[], "ConnectorPanePattern"=""} ("ClassSettings"), "ClassProviderName"=w1576, "ClassTemplateUsed"=w1577, "ClassTemplateVersion"=w1564, "ClassDescription"=w1578) -> (w1574:T3)
          n706 = call "GDSLvClass_StoreClassType.vi"("Class Refnum In"=w1579, "ClassSettings"=w1574, "error in (no error)"=w1580) -> ("Class Refnum Out"=w1561:refnum<vi>, "error out"=w1562:errorcluster)  [unwired: 15 in]
          n707 = invoke class="LVClassLibrary" method="Save"(reference=w1561, error in=w1562) -> ()  [unwired: 2 in, 4 out]
          n708 = stacked-sequence {
            tunnel: w1562 -> [_]
            frame #0 {
              n709 = Wait (ms)(milliseconds to wait=u32 5) -> ()  [unwired: 1 out]
            }
          }
          n710 = call <vilib>:"Clear Errors.vi"("error in (no error)"=w1562) -> ("error out"=w1563:errorcluster)  [unwired: 5 in, 1 out]
        }
        n711 = property on="Progress" class="LstBox (strict)"() -> ("Item Names"=w1556:string[], "Number of Rows"=w1550:u32)  [unwired: 2 in, 2 out]
        n712 = Build Array (concatenate)(w1556, "Update class info") -> (w1551:string[])
        n713 = Array Size(array=w1551) -> (size(s)=w1555:i32)
        n714 = Subtract(x=w1555, y=w1550) -> (x-y=w1554:u32)
        n715 = To Long Integer(number=w1554) -> (32bit integer=w1552:i32)
        n716 = Max & Min(x=w1552, y=0) -> (max(x,y)=w1549:i32)  [unwired: 1 out]
        n717 = property on="Progress" class="LstBox (strict)"("Item Names"=w1551, "Top Row"=w1549) -> ()  [unwired: 2 in, 2 out]
      }
    }
    n718 = call <vilib>:"Clear Errors.vi"("error in (no error)"=w20) -> ("error out"=w19:errorcluster)  [unwired: 5 in, 1 out]
    n719 = Equal?(x=w29, y="Exit") -> (x = y?=w32:bool)
    n720 = Select(t="Error", s=w19, f=w29) -> (s? t:f=w33:string)
    "State" <- w24
  }
  n721 = Unbundle By Name(w14) -> ("error"=w11:errorcluster)
  n722 = call "GDSError_ReportError.vi"("error in (no error)"=w11) -> ("error out"=w2:errorcluster)  [unwired: 18 in]
  "error out" <- w2
  n723 = property class="VI"(reference=w5, error in=w2, "Front Panel.Open"=FALSE ("Front Panel Window:Open")) -> (reference out=w3:refnum<vi>, error out=w4:errorcluster)
  n724 = Close Reference(reference=w3, error in (no error)=w4) -> ()  [unwired: 1 out]
